vi "Interface Browser.vi"(5 "Caller Window Bounds":T1, 7 "Name (\"\" to Use Uuid)":string=".interface-browser", 10 "Init State (\"Macro: Initialize\")":string="Macro: Initialize") -> ()   [LabVIEW 2017]
uses:
  <vilib>/Utility/miscctls.llb/LVRectTypeDef.ctl
  Def-FilterOption.ctl
  <vilib>/Utility/miscctls.llb/LVPoint32TypeDef.ctl
  Def-TreeData.ctl
  <vilib>/Utility/miscctls.llb/LVPointTypeDef.ctl
  AdvanceAPI/CSM - Revert Arguments-Safe String.vi
  AdvanceAPI/CSM - Break Down Multiple States String.vi
  AdvanceAPI/CSM - Compact Multiple States.vi
  AdvanceAPI/CSM - Make String Arguments Safe.vi
  AdvanceAPI/CSM - Keywords.vi
  _Polymophic/Add State(s) to Queue By BOOL(Element).vi
  _csmHelper/API/Destroy.vi
  _csmHelper/API/Stop Undo.vi
  _csmHelper/API/Open Block Diagram.vi
  _csmHelper/API/Connect Paired Tunnels.vi
  _csmHelper/API/Add State Frame.vi
  _csmHelper/API/Start Undo.vi
  _csmHelper/API/Create From VI Reference.vi
  _csmHelper/API/Open Front Panel.vi
  _Polymophic/CSM - Filter Duplicated Lines.vi
  Communicable State Machine.lvlib
  _ui/csm-ui-support.lvlib
  _csmHelper/API with lvcsm Support/CSM-Helper API with lvcsm Support.lvlib
  _interfacebrowser/interfacebrowser.lvlib
  _csmHelper/CSM-Helper.lvclass
  _csmHelper/lvcsmFile/lvcsm File Support.lvlib
  _Shared/CSM Shared.lvlib
panel:
  in  "Option:Online Only":bool
  in  "Option:All-CSM-VIs":bool
  in  "Scan Project":bool
  in  "Refresh":bool
  in  "Fast Forward":bool
  in  "Fast Reverse":bool
  in  "Skip to Beginning":bool
  in  "Skip to End":bool
  in  "Stop":bool
  in  "Play":bool
  in  "Open":bool
  in  "Refresh lvcsm Cache":bool
  in  "Filter":string
  in  "FilterOption":T2
  in  "Reset Filter":bool
  in  "MainTree":string[](tree)
  in  "Option:Sync Filter On States":bool
  in  "Zoom Factor":dbl(slide)=0.1 min=0.1 max=1.0 step=0.001 scale=0.1..1.0
  in  "Interface-Filter":enum16{"API-Only", "UserDef States", "All"}(ring)=enum."UserDef States"
  in  "CSM-States":i32[](listbox) caption="Interface"
  in  "CSM-Status":i32[](listbox) caption="Status"
  out "StateInfo@Image":string
  out "Preview":picture
  out "String":string
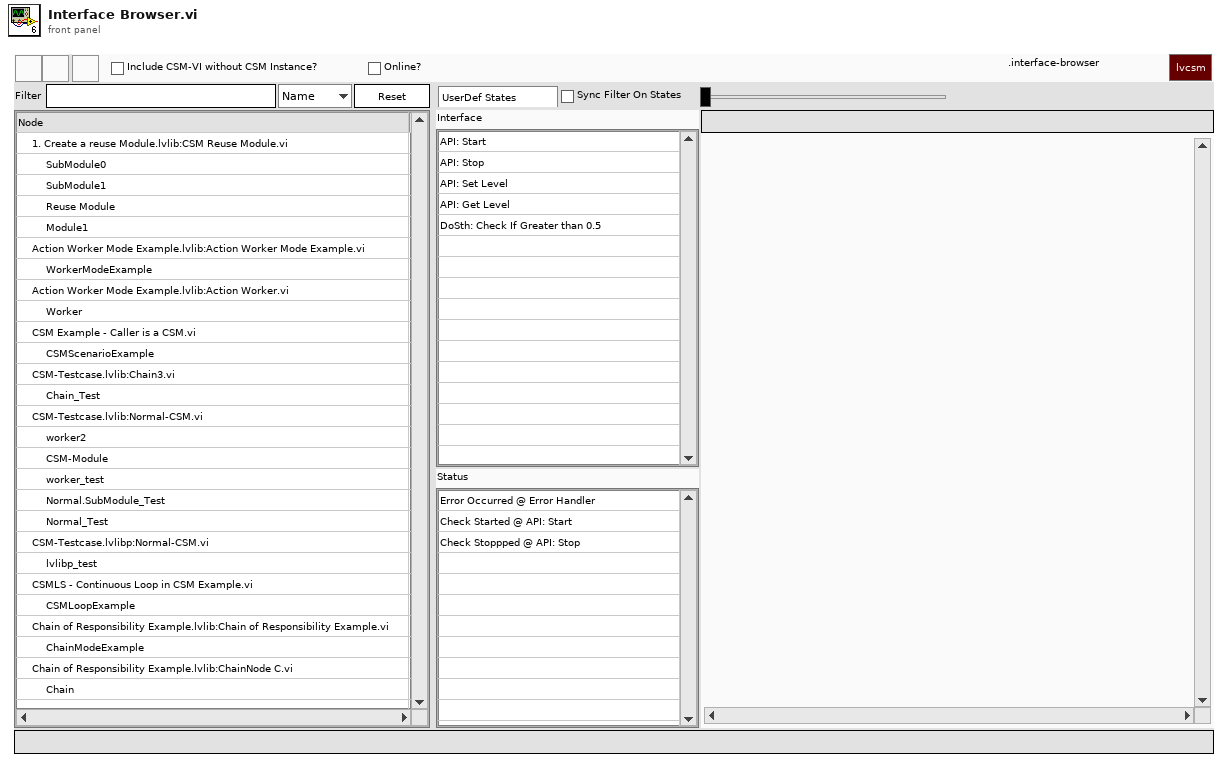
[diagram p1: front panel]
types:
  T1 = typedef "LVRectTypeDef.ctl" = cluster{"Left":i16, "Top":i16, "Right":i16, "Bottom":i16}
  T2 = typedef "Def-FilterOption.ctl" = enum16{"Name", "State"}
  T3 = enum32{"Invalid", "Standard", "Closed", "Hidden", "Minimized", "Maximized"}
  T4 = enum32{"invalid app kind", "Development System", "Run Time System", "Student Edition", "Embedded LabVIEW", "Evaluation", "Custom"}
  T5 = typedef "LVPointTypeDef.ctl" = cluster{"Horizontal":i16, "Vertical":i16}
  T6 = cluster{"Opton:All-CSM-VIs":bool, "Option:Online Only":bool}
  T7 = typedef "Communicable State Machine.lvlib/_CSM_Response Source Message.ctl" = cluster{"‘State":string, "’Arguments":string, "’Error":errorcluster}
  T8 = cluster{"Current VI Reference":refnum<vi>, "Close Panel on Exit?":bool}
  T9 = typedef "Def-TreeData.ctl" = cluster{"Type":string[], "Table":string[][]}
  T10 = cluster{"Core":cluster{"Current VI Reference":refnum<vi>, "Close Panel on Exit?":bool}, "BD-IMG":picture, "Tree":T9}
  T11 = typedef "LVPoint32TypeDef.ctl" = cluster{"Horizontal":i32, "Vertical":i32}
  T12 = cluster{"your data":bool, "PreviewMouseDown":bool, "PreviewMouseDownCoords":T11, "PreviewMouseDownOrigin":T11}
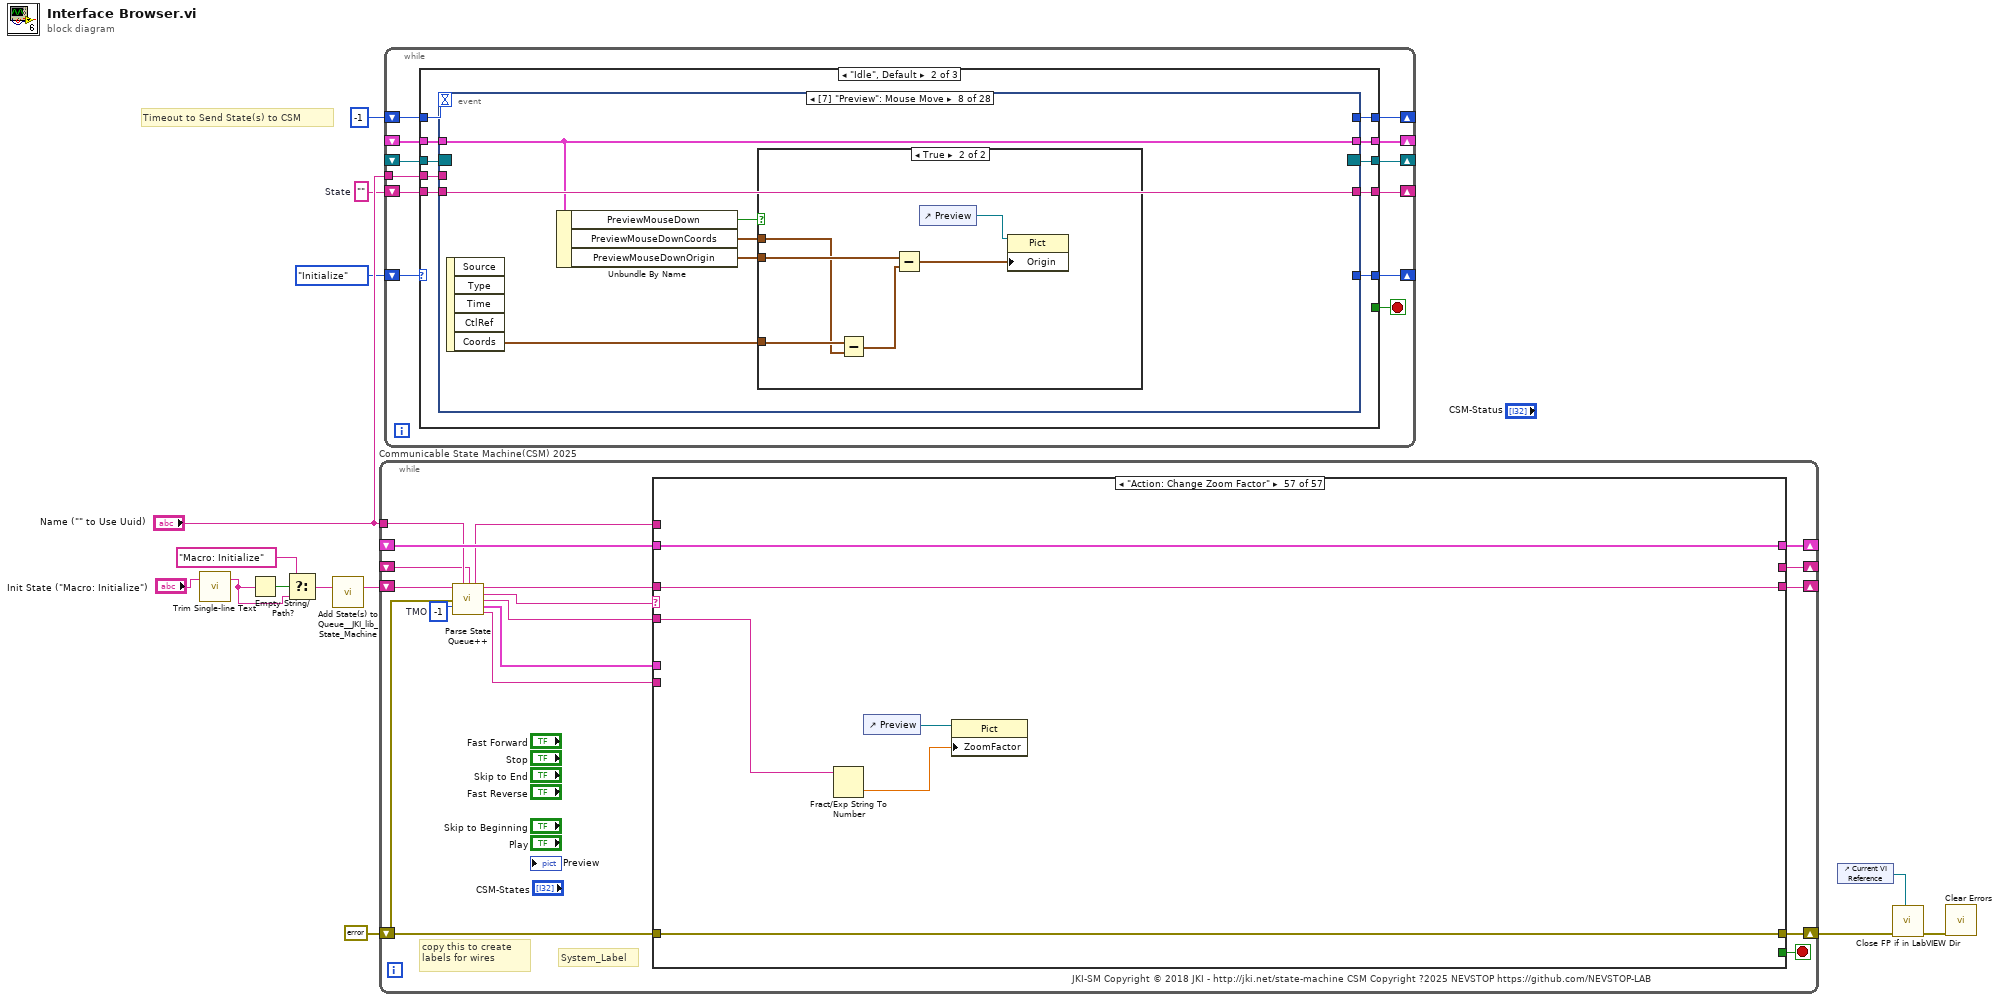
[diagram p0: block diagram]
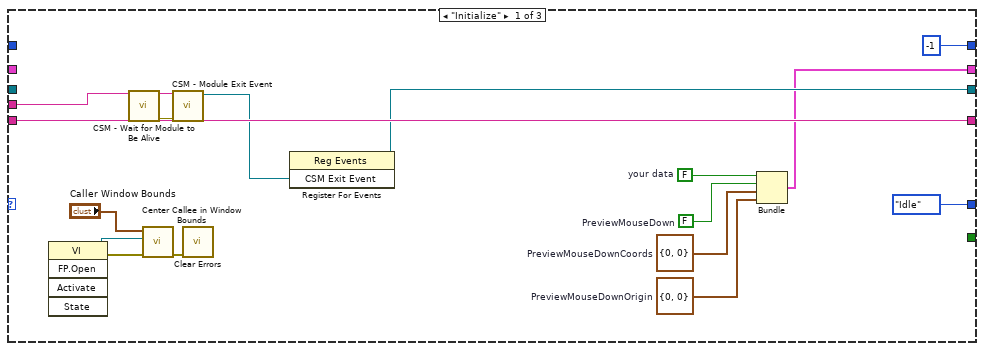
[diagram p2: hidden frame]
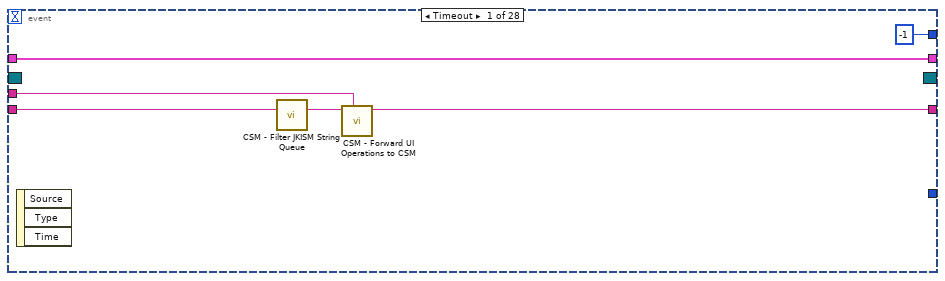
[diagram p3: hidden frame]
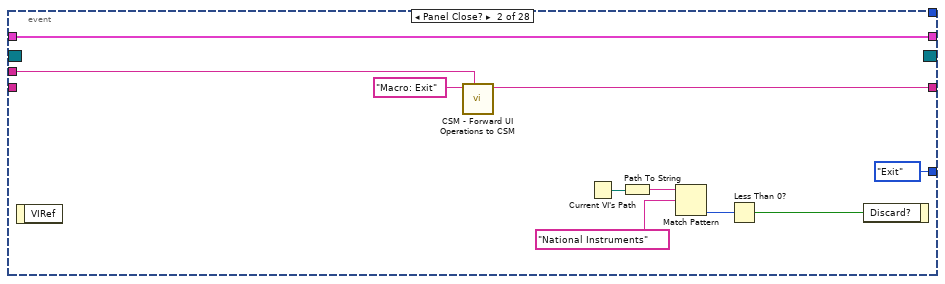
[diagram p4: hidden frame]
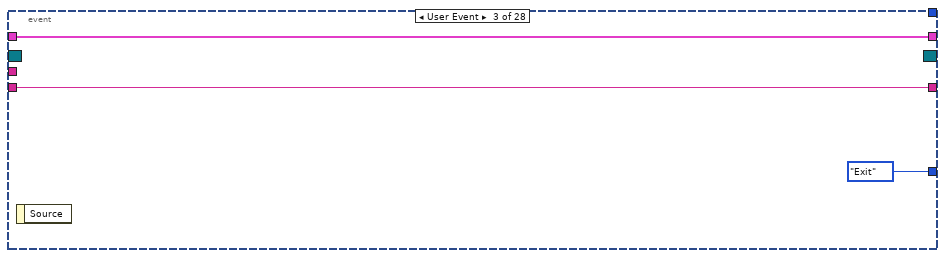
[diagram p5: hidden frame]
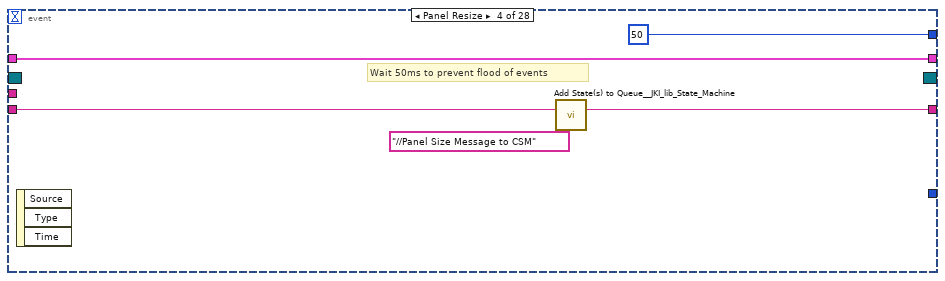
[diagram p6: hidden frame]
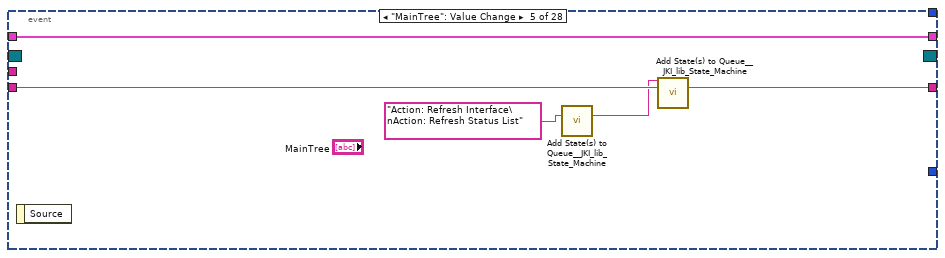
[diagram p7: hidden frame]
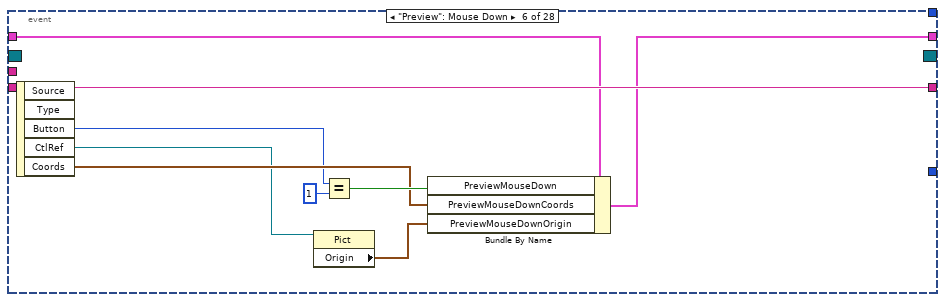
[diagram p8: hidden frame]
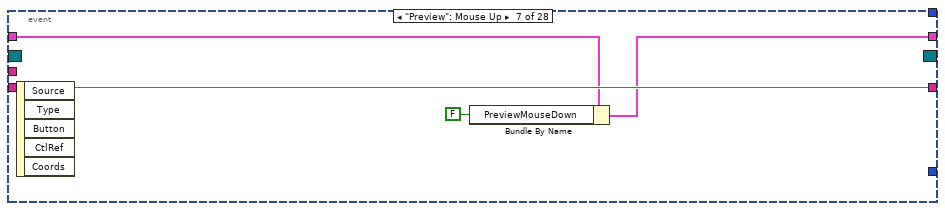
[diagram p9: hidden frame]
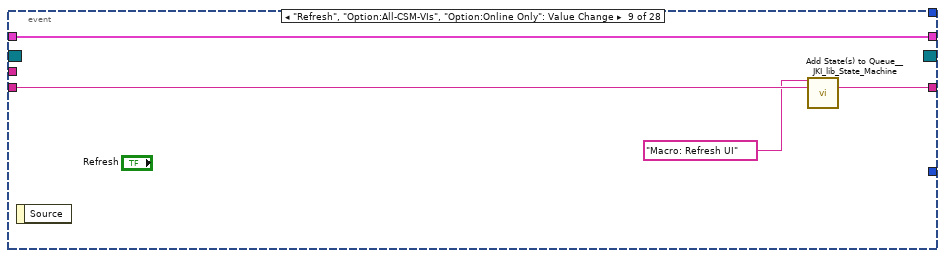
[diagram p11: hidden frame]
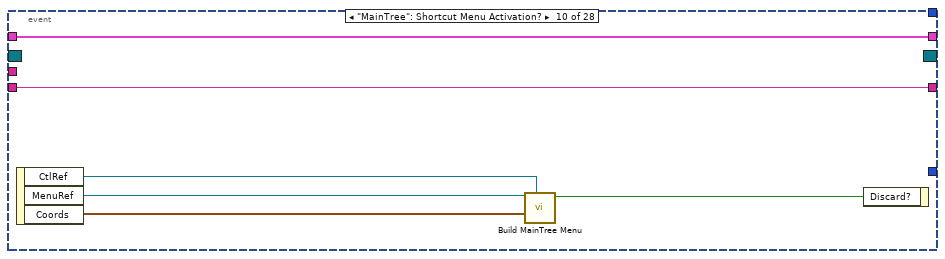
[diagram p12: hidden frame]
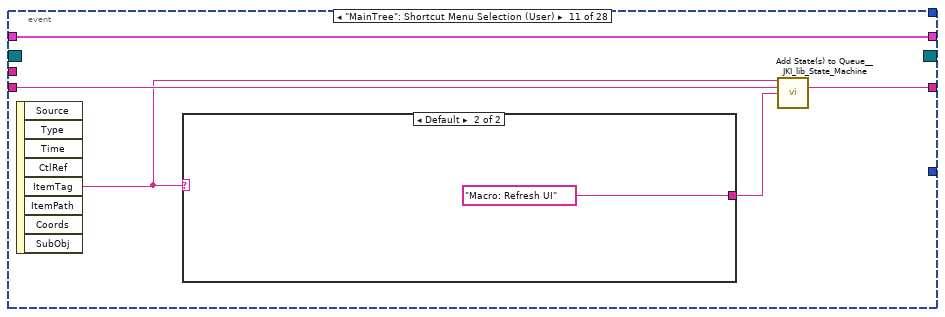
[diagram p13: hidden frame]
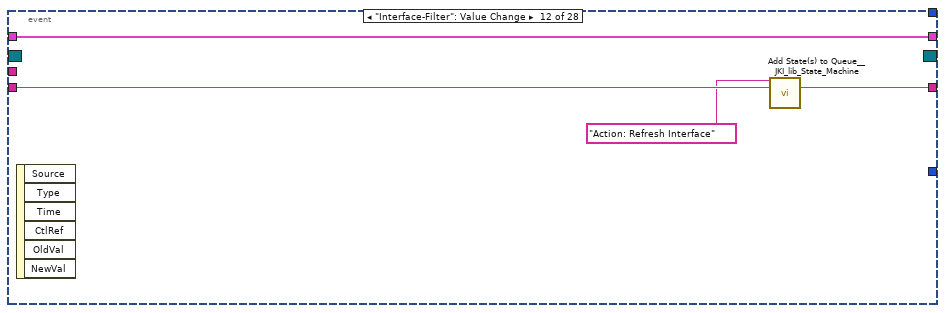
[diagram p15: hidden frame]
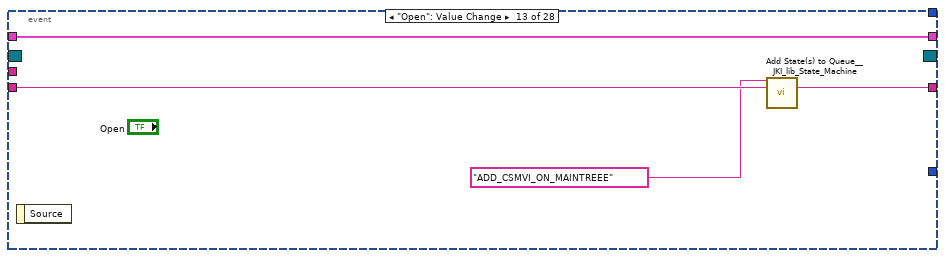
[diagram p16: hidden frame]
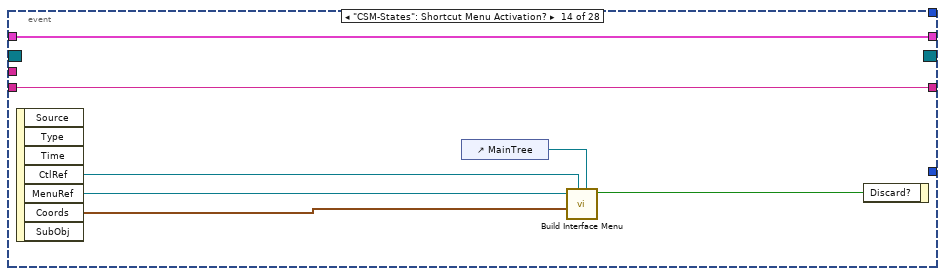
[diagram p17: hidden frame]
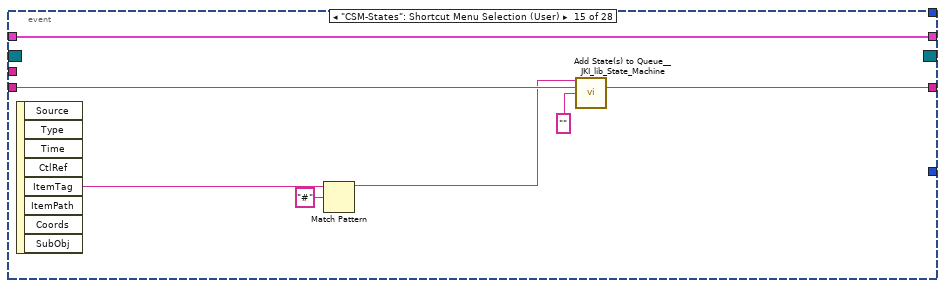
[diagram p18: hidden frame]
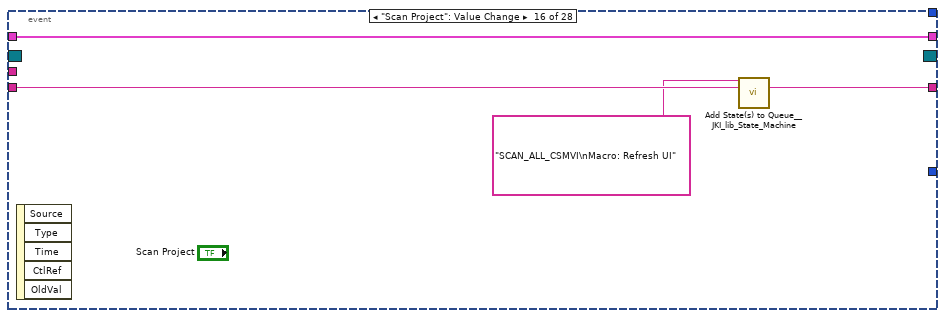
[diagram p19: hidden frame]
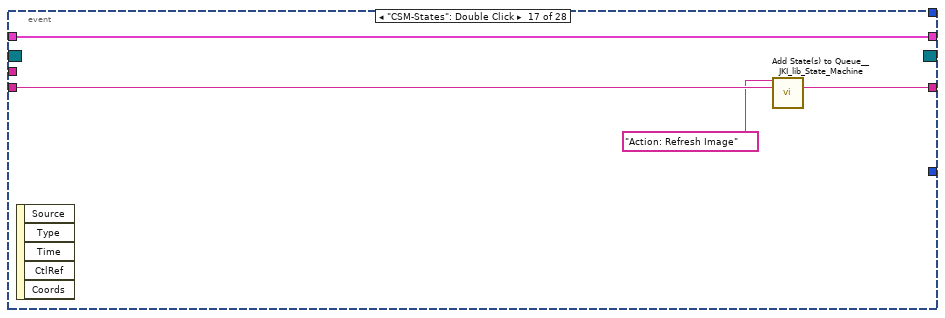
[diagram p20: hidden frame]
diagram:
  w12 = ""  # State
  # "Timeout to Send State(s) to CSM"
  n1 = call "Trim Single-line Text.vi"("single-line text"="Init State (\"Macro: Initialize\")") -> ("trimed text"=w5:string)  [unwired: 2 in]
  n2 = Empty String/Path?(string/path=w5) -> (empty?=w7:bool)
  n3 = Select(t="Macro: Initialize", s=w7, f=w5) -> (s? t:f=w6:string)
  n4 = call <vilib>:"Add State(s) to Queue__JKI_lib_State_Machine.vi"("State(s) in (\"\")"=w6) -> ("States Out"=w8:string)  [unwired: 14 in]
  n5 = while "Communicable State Machine(CSM) 2025" {
    shift-right: [w26] -> _
    shift-left: _ -> [w25]
    shift-right: [w29] -> w1
    shift-left: errorcluster {"status"=FALSE, "code"=0, "source"=""} ("error out") -> [w15]
    shift-right: [w28] -> _
    shift-left: w8 -> [w30]
    tunnel: "Name (\"\" to Use Uuid)" -> [w22]
    shift-right: [w23] -> _
    shift-left: _ -> [w17]
    stop <- w27 stop-if-true
    w24 = -1  # TMO
    # "JKI-SM Copyright © 2018 JKI - http://jki.net/state-machine CSM Copyright ?2025 NEVSTOP https://github.com/NEVSTOP-LAB"
    # "copy this to create labels for wires"
    # "System_Label"
    n6 = call "Parse State Queue++.vi"("State Queue"=w30, "Name (\"\" to Use UUID)"=w22, "Response Arguments"=w17, "Previous Error"=w15, "Dequeue (1 ms)"=w24) -> ("Name Used"=w16:string, "Remaining States"=w31:string, "Current State"=w18:string, "Arguments"=w19:string, "Additional Information"=w20:T7, "Source CSM"=w21:string)  [unwired: 5 in]
    n7 = case shown="\"Action: Change Zoom Factor\"" w18 {
      selector: w18 -> [_ _ _ w42 _ _ _ _ _ _ _ _ _ _ _ _ _ _ _ _ _ _ _ _ _ _ _ _ _ _ _ _ _ _ _ _ _ _ _ _ _ _ _ _ _ _ _ _ _ _ _ _ _ _ _ _ _]
      tunnel: w31 -> [w32 w35 w38 w46 w51 w57 w80 w86 w92 w102 w109 w121 w125 w128 w134 w149 w155 w158 w162 w166 w172 w174 w184 w198 w205 w222 w234 w255 w276 w289 w303 w317 w334 w336 w379 w404 w416 w428 w437 w458 w460 w465 w470 w482 w502 w514 w525 w536 w543 w559 w576 w615 w641 w656 w677 w697 w727]
      tunnel: w19 -> [_ _ _ _ _ w56 w76 w83 w89 w96 _ _ _ _ _ _ _ _ _ _ _ _ _ _ _ _ _ _ _ _ _ _ _ _ _ _ _ _ _ _ _ _ _ w478 w493 _ _ _ _ _ _ _ w637 _ _ _ w724]
      tunnel: w25 -> [w33 w34 w36 w44 w50 w62 w78 w84 w90 w100 w108 w115 w123 w126 _ w148 w150 w156 w160 w164 w170 w173 w183 w197 w208 w221 w233 w254 w275 w288 w302 w316 w333 w346 w384 w406 w418 w430 w436 w457 w462 w467 w469 w481 w501 w512 w523 w534 w544 w550 w574 w613 w640 w666 w686 w696 w726]
      tunnel: [_ _ _ w39 w52 errorcluster {"status"=FALSE, "code"=0, "source"=""} ("error out") w73 w81 w87 w103 _ _ _ _ _ _ w151 _ _ _ _ w175 w178 w193 _ w213 w226 w240 w256 w277 w291 w310 w332 w347 w383 w398 w412 w424 w435 w456 w463 w468 _ w472 w496 _ w516 _ w542 _ _ _ w639 _ _ w687 w728] -> w29
      tunnel: w15 -> [_ _ _ w40 w52 w60 w74 w82 w88 _ _ _ _ _ _ _ w152 _ _ _ _ w175 _ _ _ _ _ _ _ _ _ _ _ w347 _ _ _ _ _ _ w463 w468 _ _ _ _ _ _ _ _ _ _ _ _ _ _ w728]
      tunnel: [w32 w35 w37 w45 w51 w58 w79 w85 w91 w101 w109 w120 w124 w127 w133 w149 w154 w157 w161 w165 w171 w174 w184 w198 w206 w222 w234 w255 w276 w289 w303 w317 w334 w337 w380 w405 w417 w429 w437 w458 w461 w466 w470 w482 w502 w513 w524 w535 w545 w558 w575 w614 w641 w657 w678 w697 w727] -> w28
      tunnel: [_ _ _ _ _ _ TRUE _ _ _ _ _ TRUE _ _ _ _ _ _ _ _ _ _ _ _ _ _ _ _ _ _ _ _ _ _ _ _ _ _ _ _ _ _ _ _ _ _ _ _ _ _ _ _ _ _ _ _] -> w27
      tunnel: [w33 w34 w36 w44 w50 w62 w78 w84 w90 w99 w108 w119 w123 w126 w132 w148 w150 w156 w160 w164 w170 w173 w183 w197 w208 w221 w233 w254 w275 w288 w302 w316 w333 w346 w384 w406 w418 w430 w436 w457 w462 w467 w469 w481 w501 w512 w523 w533 w544 w550 w574 w613 w640 w666 w686 w696 w726] -> w26
      tunnel: w21 -> [_ _ _ _ _ w55 _ _ _ w97 _ _ _ _ _ _ _ _ _ _ _ _ _ _ _ _ _ _ _ _ _ _ _ _ _ _ _ _ w432 _ _ _ _ _ _ _ _ _ _ _ _ _ _ _ _ _ _]
      tunnel: w20 -> [_ _ _ _ _ w54 _ _ _ w98 _ _ _ _ _ _ _ _ _ _ _ _ _ _ _ _ _ _ _ _ _ _ _ _ _ _ _ _ _ _ _ _ _ _ _ _ _ _ _ _ _ _ _ _ _ _ _]
      tunnel: [_ _ _ "" w47 _ _ _ _ _ _ _ _ _ _ _ _ _ _ _ _ _ _ _ _ _ _ _ _ _ _ _ _ _ _ _ _ _ _ _ _ _ _ _ _ _ _ _ _ _ _ _ _ _ _ _ _] -> w23
      tunnel: w16 -> [_ _ _ w41 _ _ w75 _ _ _ _ _ _ _ _ _ _ _ _ _ _ _ _ _ _ _ _ _ _ _ _ _ _ _ _ _ _ _ _ _ _ _ _ _ _ _ _ _ w539 _ _ _ _ _ _ _ _]
      frame "", "Idle" {
      }
      frame "CSM Documentation" {
      }
      frame "---------- Core ----------" {
        n8 = call <vilib>:"Add State(s) to Queue__JKI_lib_State_Machine.vi"("State(s) in (\"\")"=w38) -> ("States Out"=w37:string)  [unwired: 14 in]
      }
      frame Default {
        n9 = call "CSM Unhandled State Error.vi"("error in (no error)"=w40, "Undefined State"=w42, "CSM Name"=w41) -> ("error out"=w39:errorcluster)  [unwired: 8 in]
        n10 = call <vilib>:"Add State(s) to Queue__JKI_lib_State_Machine.vi"("State(s) in (\"\")"=w46) -> ("States Out"=w45:string)  [unwired: 14 in]
      }
      frame "VI Reference" {
        n11 = Unbundle By Name(w50) -> ("Core"=w49:T8)
        n12 = Unbundle By Name(w49) -> ("Current VI Reference"=w48:refnum<vi>)
        n13 = call "CSM - Convert Data to HexStr.vi"("Variant"=w48) -> ("HEX String (0-9,A-F)"=w47:string)  [unwired: 8 in]
      }
      frame "Error Handler" {
        # "Clear error"
        n14 = case shown="Error" w60 {
          selector: w60 -> [_ w67]
          tunnel: [w66 w69] -> w59
          tunnel: w57 -> [w66 w68]
          tunnel: w56 -> [w65 _]
          tunnel: w55 -> [_ _]
          tunnel: w54 -> [_ _]
          tunnel: [w64 w67] -> w53
          frame No Error {
            n15 = call "CSM - Convert Argument to Error.vi"("Argument"=w65) -> ("Error"=w64:errorcluster)  [unwired: 4 in]
            n16 = flat-sequence {
              tunnel: w64 -> [_]
              frame #0 {
              }
            }
          }
          frame Error {
            n17 = call "CSM - Convert Error to Argument.vi"("Error"=w67) -> ("Argument"=w71:string)  [unwired: 4 in]
            n18 = call <vilib>:"Build State String with Arguments__JKI_lib_State_Machine.vi"("Arguments (\"\")"=w71, "State"="Error Occurred" ("Status with Arguments")) -> ("State with Arguments"=w70:string)  [unwired: 4 in]
            n19 = call "CSM - Broadcast Status Change.vi"("Status With Arguments"=w70, "State Queue"=w68) -> ("Remaining States"=w69:string)  [unwired: 13 in]
          }
        }
        n20 = call <vilib>:"Simple Error Handler.vi"("error in (no error)"=w53) -> ()  [unwired: 4 in, 5 out]
        n21 = call <vilib>:"Add State(s) to Queue__JKI_lib_State_Machine.vi"("State(s) in Front (\"\")"="// Post Error States", "State(s) in (\"\")"=w59) -> ("States Out"=w58:string)  [unwired: 13 in]
      }
      frame "Critical Error" {
        n22 = call "CSM Critical Error.vi"("error in (no error)"=w74, "Arugments (As Reason)"=w76, "CSM Name"=w75) -> ("error out"=w73:errorcluster)  [unwired: 8 in]
        n23 = call <vilib>:"Add State(s) to Queue__JKI_lib_State_Machine.vi"("State(s) in (\"\")"=w80) -> ("States Out"=w79:string)  [unwired: 14 in]
      }
      frame "Target Timeout Error" {
        n24 = call "CSM Target Timeout Error.vi"("error in (no error)"=w82, "Arguments (As CSM Name)"=w83) -> ("error out"=w81:errorcluster)  [unwired: 9 in]
        n25 = call <vilib>:"Add State(s) to Queue__JKI_lib_State_Machine.vi"("State(s) in (\"\")"=w86) -> ("States Out"=w85:string)  [unwired: 14 in]
      }
      frame "Target Error" {
        n26 = call "CSM Target Error.vi"("error in (no error)"=w88, "Arguments (As CSM Name)"=w89) -> ("error out"=w87:errorcluster)  [unwired: 9 in]
        n27 = call <vilib>:"Add State(s) to Queue__JKI_lib_State_Machine.vi"("State(s) in (\"\")"=w92) -> ("States Out"=w91:string)  [unwired: 14 in]
      }
      frame "Async Response", "Response" {
        n28 = Unbundle(w98) -> ("‘State"=w95:string, "’Arguments"=w94:string, "’Error"=w93:errorcluster)
        n29 = case shown="Default" w95 {
          tunnel: [w104] -> w101
          tunnel: w102 -> [w105]
          tunnel: [w107] -> w99
          tunnel: w100 -> [w107]
          tunnel: [w106] -> w103
          tunnel: w93 -> [w106]
          tunnel: w97 -> [_]
          tunnel: w96 -> [_]
          tunnel: w94 -> [_]
          frame Default {
            n30 = call <vilib>:"Add State(s) to Queue__JKI_lib_State_Machine.vi"("State(s) in (\"\")"=w105) -> ("States Out"=w104:string)  [unwired: 14 in]
          }
        }
      }
      frame "Async Message Posted" {
      }
      frame "Initialize Core Data" {
        # "originally closed?"
        # "exe?"
        # "If panel starts closed or is an EXE, then close it when we exit"
        n31 = control-ref of="Current VI Reference"() -> (w113:refnum<vi>)
        n32 = property class="VI"() -> ("FP.State"=w112:T3)  [unwired: 2 in, 2 out]
        n33 = property class="App"() -> ("App.Kind"=w118:T4)  [unwired: 2 in, 2 out]
        n34 = Equal?(x=w112, y=T3."Closed" ("Front Panel Window:State")) -> (x = y?=w110:bool)
        n35 = Equal?(x=w118, y=T4."Run Time System" ("Application:Kind")) -> (x = y?=w116:bool)
        n36 = Or(x=w110, y=w116) -> (x .or. y?=w114:bool)
        n37 = Bundle By Name(cluster=w115, "Core.Current VI Reference"=w113, "Core.Close Panel on Exit?"=w114) -> (w119:T10)
        n38 = call <vilib>:"Add State(s) to Queue__JKI_lib_State_Machine.vi"("State(s) in (\"\")"=w121) -> ("States Out"=w120:string)  [unwired: 14 in]
      }
      frame "Exit" {
        n39 = call <vilib>:"Add State(s) to Queue__JKI_lib_State_Machine.vi"("State(s) in (\"\")"=w125) -> ("States Out"=w124:string)  [unwired: 14 in]
      }
      frame "---------- Data ----------" {
        n40 = call <vilib>:"Add State(s) to Queue__JKI_lib_State_Machine.vi"("State(s) in (\"\")"=w128) -> ("States Out"=w127:string)  [unwired: 14 in]
      }
      frame "Data: Initialize" {
        w129 = T9 {"Type"=[], "Table"=[]}  # Tree
        w130 = picture data[5B]  # BD-IMG
        w131 = T8 {"Current VI Reference"=refnum, "Close Panel on Exit?"=FALSE}  # Core
        n41 = Bundle("Core"=w131, "BD-IMG"=w130, "Tree"=w129) -> (w132:T10)  [unwired: 1 in]
        n42 = call <vilib>:"Add State(s) to Queue__JKI_lib_State_Machine.vi"("State(s) in (\"\")"=w134) -> ("States Out"=w133:string)  [unwired: 14 in]
      }
      frame "Data: Update Indicators" {
        n43 = property class="App"() -> ("Project.ActiveProject"=w144:refnum<vi>)  [unwired: 2 in, 2 out]
        n44 = property class="Project"(reference=w144) -> ("Path"=w145:path)  [unwired: 1 in, 2 out]
        n45 = Strip Path(path=w145) -> (stripped path=w141:path)  [unwired: 1 out]
        n46 = local write "Preview"(picture data[5B] ("2D Picture 2")) -> ()
        n47 = local write "FilterOption"(Def-FilterOption."Name" ("FilterOption")) -> ()
        n48 = property on="Preview" class="Pict"("Origin"=T5 {"Horizontal"=0, "Vertical"=0}) -> ()  [unwired: 2 in, 2 out]
        n49 = Path To String(path=w141) -> (string=w140:string)
        n50 = call <vilib>:"Build State String with Arguments__JKI_lib_State_Machine.vi"("Arguments (\"\")"=w140, "State"="Interface Browser (CSM) ") -> ("State with Arguments"=w143:string)  [unwired: 4 in]
        n51 = property on="CSM-Status" class="LstBox (strict)"("Item Names"=string[] []) -> ()  [unwired: 2 in, 2 out]
        n52 = local write "Option:Sync Filter On States"(TRUE ("Option:Sync Filter On States")) -> ()
        n53 = local write "Zoom Factor"(0.7 ("Zoom Factor")) -> ()
        n54 = local write "Filter"("" ("Filter")) -> ()
        n55 = property class="VI"("Front Panel.Title"=w143) -> ()  [unwired: 2 in, 2 out]
      }
      frame "Data: Cleanup" {
        n56 = Unbundle By Name(w150) -> ("Core.Current VI Reference"=w153:refnum<vi>)
        n57 = Close Reference(reference=w153, error in (no error)=w152) -> (error out=w151:errorcluster)
        n58 = call <vilib>:"Add State(s) to Queue__JKI_lib_State_Machine.vi"("State(s) in (\"\")"=w155) -> ("States Out"=w154:string)  [unwired: 14 in]
      }
      frame "---------- Macro ----------" {
        n59 = call <vilib>:"Add State(s) to Queue__JKI_lib_State_Machine.vi"("State(s) in (\"\")"=w158) -> ("States Out"=w157:string)  [unwired: 14 in]
      }
      frame "Macro: Initialize" {
        n60 = call <vilib>:"Add State(s) to Queue__JKI_lib_State_Machine.vi"("State(s) in Front (\"\")"="Data: Initialize\nInitialize Core Data\nData: Update Indicators\nMacro: Refresh UI", "State(s) in (\"\")"=w162) -> ("States Out"=w161:string)  [unwired: 13 in]
      }
      frame "Macro: Refresh UI" {
        n61 = call <vilib>:"Add State(s) to Queue__JKI_lib_State_Machine.vi"("State(s) in Front (\"\")"="Action: Refresh(CSM-VI mode)\nAction: Refresh Symbol\nAction: Refresh Interface\nAction: Refresh Status List\nAction: Refresh Image\n", "State(s) in (\"\")"=w166) -> ("States Out"=w165:string)  [unwired: 13 in]
      }
      frame "Macro: Exit" {
        n62 = call <vilib>:"Add State(s) to Queue__JKI_lib_State_Machine.vi"("State(s) in Front (\"\")"="//Exit Sub-Modules ", "State(s) at Back (\"\")"="Data: Cleanup\nExit") -> ("States Out"=w168:string)  [unwired: 13 in]
        n63 = call <vilib>:"Add State(s) to Queue__JKI_lib_State_Machine.vi"("State(s) in Front (\"\")"=w168, "State(s) in (\"\")"=w172) -> ("States Out"=w171:string)  [unwired: 13 in]
      }
      frame "------ Menu Handler ------" {
      }
      frame "ADD_CSM_ON_CSMVI" {
        n64 = control-ref of="MainTree"() -> (w182:refnum<vi>)
        n65 = property class="Tree (strict)"(reference=w182) -> ("Value"=w181:string[])  [unwired: 1 in, 2 out]
        n66 = call "CSM Module Name"() -> ("CSM Module"=w179:string, "OK"=w177:bool)  [unwired: 17 in, 1 out]
        n67 = Index Array(array=w181) -> (element=w180:string)  [unwired: 1 in]
        n68 = call <vilib>:"Trim Whitespace.vi"("string"=w179) -> ("trimmed string"=w176:string)  [unwired: 1 in]
        n69 = case shown="True" w177 {
          tunnel: w180 -> [_ w187]
          tunnel: w176 -> [_ w186]
          tunnel: [_ w185] -> w178
          frame False {
          }
          frame True {
            n70 = call "Add CSM Module.vi"("CSM-VI"=w187, "CSM Name"=w186) -> ("error out"=w185:errorcluster)  [unwired: 9 in]
          }
        }
      }
      frame "ADD_CSM_ON_CSM" {
        n71 = control-ref of="MainTree"() -> (w196:refnum<vi>)
        n72 = property class="Tree (strict)"(reference=w196) -> ("Value"=w195:string[])  [unwired: 1 in, 2 out]
        n73 = Index Array(array=w195) -> (element=w190:string)  [unwired: 1 in]
        n74 = call "CSM Module Name2"() -> ("CSM Module"=w194:string, "OK"=w192:bool)  [unwired: 17 in, 1 out]
        n75 = Match Pattern(string=w190, regular expression="/") -> (before substring=w189:string)  [unwired: 1 in, 3 out]
        n76 = call <vilib>:"Trim Whitespace.vi"("string"=w194) -> ("trimmed string"=w191:string)  [unwired: 1 in]
        n77 = case shown="True" w192 {
          tunnel: w189 -> [_ w201]
          tunnel: w191 -> [_ w200]
          tunnel: [_ w199] -> w193
          frame False {
          }
          frame True {
            n78 = call "Add CSM Module.vi"("CSM-VI"=w201, "CSM Name"=w200) -> ("error out"=w199:errorcluster)  [unwired: 9 in]
          }
        }
      }
      frame "ADD_CSMVI_ON_MAINTREEE" {
        n79 = call "File Dialog"("pattern (all files)"="*.vi") -> ("selected path"=w203:path, "error out"=w204:errorcluster)  [unwired: 11 in, 2 out]
        n80 = case shown="Error" w204 {
          selector: w204 -> [w211 _]
          tunnel: w203 -> [w212 _]
          tunnel: ["Macro: Refresh UI" ("State(s) in Front (\"\")") _] -> w202
          frame No Error {
            n81 = call "Add CSM-VI.vi"("error in (no error)"=w211, "CSM-VI"=w212) -> ("error out"=w209:errorcluster)  [unwired: 9 in]
            n82 = call <vilib>:"Simple Error Handler.vi"("error in (no error)"=w209) -> ()  [unwired: 4 in, 5 out]
          }
          frame Error {
          }
        }
        n83 = call <vilib>:"Add State(s) to Queue__JKI_lib_State_Machine.vi"("State(s) in Front (\"\")"=w202, "State(s) in (\"\")"=w205) -> ("States Out"=w206:string)  [unwired: 13 in]
      }
      frame "RM_CSM_ON_CSM" {
        n84 = control-ref of="MainTree"() -> (w220:refnum<vi>)
        n85 = property class="Tree (strict)"(reference=w220) -> ("Value"=w219:string[])  [unwired: 1 in, 2 out]
        n86 = Index Array(array=w219) -> (element=w218:string)  [unwired: 1 in]
        n87 = Two Button Dialog(message="Are you sure to remove it?") -> (T button?=w214:bool)  [unwired: 2 in]
        n88 = Match Pattern(string=w218, regular expression="/") -> (after substring=w215:string)  [unwired: 1 in, 3 out]
        n89 = case shown="True" w214 {
          tunnel: w215 -> [_ w224]
          tunnel: [_ w223] -> w213
          frame False {
          }
          frame True {
            n90 = call "Delete CSM Module.vi"("CSM Name"=w224) -> ("error out"=w223:errorcluster)  [unwired: 10 in]
          }
        }
      }
      frame "RM_CSMVI_ON_CSMVI" {
        n91 = control-ref of="MainTree"() -> (w232:refnum<vi>)
        n92 = property class="Tree (strict)"(reference=w232) -> ("Value"=w231:string[])  [unwired: 1 in, 2 out]
        n93 = Index Array(array=w231) -> (element=w230:string)  [unwired: 1 in]
        n94 = Two Button Dialog(message="Are you sure to remove it?") -> (T button?=w227:bool)  [unwired: 2 in]
        n95 = Match Pattern(string=w230, regular expression="/") -> (before substring=w225:string)  [unwired: 1 in, 3 out]
        n96 = case shown="True" w227 {
          tunnel: w225 -> [_ w236]
          tunnel: [_ w235] -> w226
          frame False {
          }
          frame True {
            n97 = call "Delete CSM-VI.vi"("CSM Name"=w236) -> ("error out"=w235:errorcluster)  [unwired: 10 in]
          }
        }
      }
      frame "OPEN_CSMVI_ON_CSM", "OPEN_CSMVI_ON_CSMVI" {
        n98 = control-ref of="MainTree"() -> (w253:refnum<vi>)
        n99 = property class="Tree (strict)"(reference=w253) -> ("Value"=w252:string[])  [unwired: 1 in, 2 out]
        n100 = Index Array(array=w252) -> (element=w251:string)  [unwired: 1 in]
        n101 = Match Pattern(string=w251, regular expression="/") -> (before substring=w249:string)  [unwired: 1 in, 3 out]
        n102 = call "Read CSM-VI Info.vi"("CSM Name"=w249) -> ("Cluster 2"=w248:cluster{"Path":path})  [unwired: 9 in, 1 out]
        n103 = Unbundle By Name(w248) -> ("Path"=w238:path)
        n104 = Path To String(path=w238) -> (string=w237:string)
        n105 = call "lvcsm String to Path.vi"("Common Path"=w237) -> ("Path"=w239:path)  [unwired: 10 in]
        n106 = Open VI Reference(vi path=w239, options=2) -> (vi reference=w246:refnum<vi>, error out=w245:errorcluster)  [unwired: 4 in]
        n107 = call-poly "CSM-Helper API.vi"("error in (no error)"=w245, "VI"=w246) -> ("error out"=w243:errorcluster, "CSM-Helper.lvclass"=w244:refnum<class "CSM-Helper.lvclass">)  [unwired: 8 in]
        n108 = call-poly "CSM-Helper API.vi"("error in (no error)"=w243, "CSM-Helper in"=w244) -> ("error out"=w241:errorcluster, "CSM-Helper out"=w242:refnum<class "CSM-Helper.lvclass">)  [unwired: 8 in]
        n109 = call-poly "CSM-Helper API.vi"("error in (no error)"=w241, "CSM-Helper in"=w242) -> ("error out"=w240:errorcluster)  [unwired: 8 in, 1 out]
      }
      frame "EXPLORER_TO_FOLDER_ON_CSMVI" {
        n110 = control-ref of="MainTree"() -> (w274:refnum<vi>)
        n111 = property class="Tree (strict)"(reference=w274) -> ("Value"=w273:string[])  [unwired: 1 in, 2 out]
        n112 = Index Array(array=w273) -> (element=w272:string)  [unwired: 1 in]
        n113 = Match Pattern(string=w272, regular expression="/") -> (before substring=w270:string)  [unwired: 1 in, 3 out]
        n114 = call "Read CSM-VI Info.vi"("CSM Name"=w270) -> ("Cluster 2"=w269:cluster{"Path":path})  [unwired: 9 in, 1 out]
        n115 = Unbundle By Name(w269) -> ("Path"=w268:path)
        n116 = Path To String(path=w268) -> (string=w267:string)
        n117 = call "lvcsm String to Path.vi"("Common Path"=w267) -> ("Path"=w258:path)  [unwired: 10 in]
        n118 = File/Directory Info(path=w258) -> (directory=w264:bool, error out=w263:errorcluster)  [unwired: 1 in, 5 out]
        n119 = Compound Arithmetic op=OR(TRUE ("value"), invert w264) -> (w262:bool)
        n120 = Select(t="/select," ("format string"), s=w262, f="") -> (s? t:f=w261:string)
        n121 = Format Into String(format string="explorer %s\"%s\"", w261, w258) -> (resulting string=w265:string)  [unwired: 2 in, 1 out]
        n122 = call <vilib>:"System Exec.vi"("error in (no error)"=w263, "command line"=w265) -> ("error out"=w256:errorcluster)  [unwired: 6 in, 3 out]
      }
      frame "COPY_FULL_PATH_TO_CLIPBOARD" {
        n123 = control-ref of="MainTree"() -> (w287:refnum<vi>)
        n124 = property class="Tree (strict)"(reference=w287) -> ("Value"=w286:string[])  [unwired: 1 in, 2 out]
        n125 = Index Array(array=w286) -> (element=w285:string)  [unwired: 1 in]
        n126 = Match Pattern(string=w285, regular expression="/") -> (before substring=w283:string)  [unwired: 1 in, 3 out]
        n127 = call "Read CSM-VI Info.vi"("CSM Name"=w283) -> ("Cluster 2"=w282:cluster{"Path":path})  [unwired: 9 in, 1 out]
        n128 = Unbundle By Name(w282) -> ("Path"=w281:path)
        n129 = Path To String(path=w281) -> (string=w280:string)
        n130 = call "lvcsm String to Path.vi"("Common Path"=w280) -> ("Path"=w279:path)  [unwired: 10 in]
        n131 = Path To String(path=w279) -> (string=w278:string)
        n132 = invoke class="App" method="Clipboard.Write"("Param 0"=w278) -> (error out=w277:errorcluster)  [unwired: 3 in, 3 out]
      }
      frame "COPY_CNT_FOLDER_TO_CLIPBOARD" {
        n133 = control-ref of="MainTree"() -> (w301:refnum<vi>)
        n134 = property class="Tree (strict)"(reference=w301) -> ("Value"=w300:string[])  [unwired: 1 in, 2 out]
        n135 = Index Array(array=w300) -> (element=w299:string)  [unwired: 1 in]
        n136 = Match Pattern(string=w299, regular expression="/") -> (before substring=w297:string)  [unwired: 1 in, 3 out]
        n137 = call "Read CSM-VI Info.vi"("CSM Name"=w297) -> ("Cluster 2"=w296:cluster{"Path":path})  [unwired: 9 in, 1 out]
        n138 = Unbundle By Name(w296) -> ("Path"=w295:path)
        n139 = Path To String(path=w295) -> (string=w294:string)
        n140 = call "lvcsm String to Path.vi"("Common Path"=w294) -> ("Path"=w293:path)  [unwired: 10 in]
        n141 = Strip Path(path=w293) -> (stripped path=w290:path)  [unwired: 1 out]
        n142 = Path To String(path=w290) -> (string=w292:string)
        n143 = invoke class="App" method="Clipboard.Write"("Param 0"=w292) -> (error out=w291:errorcluster)  [unwired: 3 in, 3 out]
      }
      frame "GOTO_ON_CSMSTATE" {
        n144 = control-ref of="MainTree"() -> (w309:refnum<vi>)
        n145 = control-ref of="CSM-States"() -> (w314:refnum<vi>)
        n146 = property class="LstBox (strict)"(reference=w314) -> ("Item Names"=w315:string[], "Value"=w313:i32[])  [unwired: 1 in, 2 out]
        n147 = property class="Tree (strict)"(reference=w309) -> ("Value"=w308:string[])  [unwired: 1 in, 2 out]
        n148 = Index Array(array=w313) -> (element=w312:i32)  [unwired: 1 in]
        n149 = Index Array(array=w308) -> (element=w307:string)  [unwired: 1 in]
        n150 = Index Array(array=w315, index=w312) -> (element=w311:string)
        n151 = Match Pattern(string=w307, regular expression="/") -> (before substring=w305:string)  [unwired: 1 in, 3 out]
        n152 = call "Jump to CSM State.vi"("Type"=enum16{"CSM", "CSM-VI"}."CSM-VI", "State"=w311, "Name"=w305) -> ("error out"=w310:errorcluster)  [unwired: 8 in]
      }
      frame "GOTO_ON_CSMSTATUS" {
        (unwired) "@" ("string")
        n153 = control-ref of="CSM-Status"() -> (w322:refnum<vi>)
        n154 = property class="LstBox (strict)"(reference=w322) -> ("Item Names"=w325:string[], "Value"=w324:i32[])  [unwired: 1 in, 2 out]
        n155 = control-ref of="MainTree"() -> (w331:refnum<vi>)
        n156 = Index Array(array=w324) -> (element=w323:i32)  [unwired: 1 in]
        n157 = property class="Tree (strict)"(reference=w331) -> ("Value"=w330:string[])  [unwired: 1 in, 2 out]
        n158 = Index Array(array=w325, index=w323) -> (element=w321:string)
        n159 = Match Pattern(string=w321, regular expression="@") -> (after substring=w320:string)  [unwired: 1 in, 3 out]
        n160 = Index Array(array=w330) -> (element=w329:string)  [unwired: 1 in]
        n161 = call <vilib>:"Trim Whitespace.vi"("string"=w320) -> ("trimmed string"=w318:string)  [unwired: 1 in]
        n162 = Match Pattern(string=w329, regular expression="/") -> (before substring=w327:string)  [unwired: 1 in, 3 out]
        n163 = call "Jump to CSM State.vi"("Type"=enum16{"CSM", "CSM-VI"}."CSM-VI", "State"=w318, "Name"=w327) -> ("error out"=w332:errorcluster)  [unwired: 8 in]
      }
      frame "ADD_STATE_ON_CSMSTATE" {
        n164 = call "Add State"() -> ("State Name"=w345:string, "OK"=w338:bool, "error out"=w340:errorcluster)  [unwired: 17 in]
        n165 = Not(x=w340) -> (.not. x?=w341:bool)
        n166 = Empty String/Path?(string/path=w345) -> (empty?=w343:bool)
        n167 = And(x=w341, y=w338) -> (x .and. y?=w339:bool)
        n168 = Not(x=w343) -> (.not. x?=w344:bool)
        n169 = And(x=w344, y=w339) -> (x .and. y?=w342:bool)
        n170 = case shown="True" w342 {
          tunnel: w345 -> [_ w362]
          tunnel: [_ "RESCAN_INTERFACE_ON_CSMVI\nMacro: Refresh UI" ("State(s) in Front (\"\")")] -> w335
          frame False {
          }
          frame True {
            n171 = control-ref of="MainTree"() -> (w375:refnum<vi>)
            n172 = control-ref of="CSM-States"() -> (w376:refnum<vi>)
            n173 = property class="LstBox (strict)"(reference=w376) -> ("Item Names"=w377:string[])  [unwired: 1 in, 2 out]
            n174 = property class="Tree (strict)"(reference=w375) -> ("Value"=w374:string[])  [unwired: 1 in, 2 out]
            n175 = Index Array(array=w377) -> ()  [unwired: 1 in, 1 out]
            n176 = Index Array(array=w374) -> (element=w373:string)  [unwired: 1 in]
            n177 = Match Pattern(string=w373, regular expression="/") -> (before substring=w368:string)  [unwired: 1 in, 3 out]
            n178 = call "Read CSM-VI Info.vi"("CSM Name"=w368) -> ("error out"=w364:errorcluster, "Cluster 2"=w369:cluster{"Path":path})  [unwired: 9 in]
            n179 = Unbundle By Name(w369) -> ("Path"=w371:path)
            n180 = Path To String(path=w371) -> (string=w370:string)
            n181 = call "lvcsm String to Path.vi"("Common Path"=w370) -> ("Path"=w365:path)  [unwired: 10 in]
            n182 = Open VI Reference(vi path=w365, options=2, error in (no error)=w364) -> (vi reference=w366:refnum<vi>, error out=w367:errorcluster)  [unwired: 3 in]
            n183 = call-poly "CSM-Helper API.vi"("error in (no error)"=w367, "VI"=w366) -> ("error out"=w361:errorcluster, "CSM-Helper.lvclass"=w360:refnum<class "CSM-Helper.lvclass">)  [unwired: 8 in]
            n184 = call-poly "CSM-Helper API.vi"("error in (no error)"=w361, "CSM-Helper in"=w360) -> ("error out"=w359:errorcluster, "CSM-Helper out"=w358:refnum<class "CSM-Helper.lvclass">)  [unwired: 8 in]
            n185 = call-poly "CSM-Helper API.vi"("error in (no error)"=w359, "element"=w362, "CSM-Helper in"=w358) -> ("error out"=w351:errorcluster, "CSM-Helper out"=w350:refnum<class "CSM-Helper.lvclass">)  [unwired: 6 in, 1 out]
            n186 = call-poly "CSM-Helper API.vi"("error in (no error)"=w351, "CSM-Helper in"=w350) -> ("error out"=w348:errorcluster, "CSM-Helper out"=w349:refnum<class "CSM-Helper.lvclass">)  [unwired: 8 in]
            n187 = call-poly "CSM-Helper API.vi"("error in (no error)"=w348, "CSM-Helper in"=w349) -> ("error out"=w352:errorcluster, "CSM-Helper out"=w353:refnum<class "CSM-Helper.lvclass">)  [unwired: 8 in]
            n188 = call-poly "CSM-Helper API.vi"("error in (no error)"=w352, "CSM-Helper in"=w353) -> ("error out"=w357:errorcluster, "CSM-Helper out"=w356:refnum<class "CSM-Helper.lvclass">)  [unwired: 8 in]
            n189 = call-poly "CSM-Helper API.vi"("error in (no error)"=w357, "CSM-Helper in"=w356) -> ("error out"=w355:errorcluster)  [unwired: 8 in, 1 out]
            n190 = call <vilib>:"Simple Error Handler.vi"("error in (no error)"=w355) -> ()  [unwired: 4 in, 5 out]
          }
        }
        n191 = call <vilib>:"Add State(s) to Queue__JKI_lib_State_Machine.vi"("State(s) in Front (\"\")"=w335, "State(s) in (\"\")"=w336) -> ("States Out"=w337:string)  [unwired: 13 in]
      }
      frame "DELETE_STATE_ON_CSMSTATE" {
        n192 = Two Button Dialog(message="Are you sure?") -> (T button?=w381:bool)  [unwired: 2 in]
        n193 = case shown="True" w381 {
          tunnel: [_ w397] -> w383
          tunnel: [_ "RESCAN_INTERFACE_ON_CSMVI\nMacro: Refresh UI" ("State(s) in Front (\"\")")] -> w378
          frame False {
          }
          frame True {
            n194 = control-ref of="MainTree"() -> (w391:refnum<vi>)
            n195 = control-ref of="CSM-States"() -> (w395:refnum<vi>)
            n196 = property class="LstBox (strict)"(reference=w395) -> ("Item Names"=w396:string[], "Value"=w394:i32[])  [unwired: 1 in, 2 out]
            n197 = property class="Tree (strict)"(reference=w391) -> ("Value"=w390:string[])  [unwired: 1 in, 2 out]
            n198 = Index Array(array=w394) -> (element=w393:i32)  [unwired: 1 in]
            n199 = Index Array(array=w390) -> (element=w389:string)  [unwired: 1 in]
            n200 = Index Array(array=w396, index=w393) -> (element=w392:string)
            n201 = Match Pattern(string=w389, regular expression="/") -> (before substring=w387:string)  [unwired: 1 in, 3 out]
            n202 = call "Delete CSM State.vi"("Type"=enum16{"CSM", "CSM-VI"}."CSM-VI", "State"=w392, "Name"=w387) -> ("Error Out"=w397:errorcluster)  [unwired: 8 in]
          }
        }
        n203 = call <vilib>:"Add State(s) to Queue__JKI_lib_State_Machine.vi"("State(s) in Front (\"\")"=w378, "State(s) in (\"\")"=w379) -> ("States Out"=w380:string)  [unwired: 13 in]
      }
      frame "COPY_TO_CLIPBOARD_ON_CSMSTATE" {
        n204 = control-ref of="CSM-States"() -> (w402:refnum<vi>)
        n205 = property class="LstBox (strict)"(reference=w402) -> ("Item Names"=w403:string[], "Value"=w401:i32[])  [unwired: 1 in, 2 out]
        n206 = Index Array(array=w401) -> (element=w400:i32)  [unwired: 1 in]
        n207 = Index Array(array=w403, index=w400) -> (element=w399:string)
        n208 = invoke class="App" method="Clipboard.Write"("Param 0"=w399) -> (error out=w398:errorcluster)  [unwired: 3 in, 3 out]
        n209 = call <vilib>:"Add State(s) to Queue__JKI_lib_State_Machine.vi"("State(s) in (\"\")"=w404) -> ("States Out"=w405:string)  [unwired: 14 in]
      }
      frame "COPY_STATUS_TO_CLIPBOARD_ON_CSMSTATUS" {
        n210 = control-ref of="CSM-Status"() -> (w411:refnum<vi>)
        n211 = property class="LstBox (strict)"(reference=w411) -> ("Item Names"=w415:string[], "Value"=w414:i32[])  [unwired: 1 in, 2 out]
        n212 = Index Array(array=w414) -> (element=w413:i32)  [unwired: 1 in]
        n213 = Index Array(array=w415, index=w413) -> (element=w410:string)
        n214 = Match Pattern(string=w410, regular expression="@") -> (before substring=w408:string)  [unwired: 1 in, 3 out]
        n215 = call <vilib>:"Trim Whitespace.vi"("string"=w408) -> ("trimmed string"=w407:string)  [unwired: 1 in]
        n216 = invoke class="App" method="Clipboard.Write"("Param 0"=w407) -> (error out=w412:errorcluster)  [unwired: 3 in, 3 out]
        n217 = call <vilib>:"Add State(s) to Queue__JKI_lib_State_Machine.vi"("State(s) in (\"\")"=w416) -> ("States Out"=w417:string)  [unwired: 14 in]
      }
      frame "COPY_STATE_TO_CLIPBOARD_ON_CSMSTATUS" {
        n218 = control-ref of="CSM-Status"() -> (w423:refnum<vi>)
        n219 = property class="LstBox (strict)"(reference=w423) -> ("Item Names"=w427:string[], "Value"=w426:i32[])  [unwired: 1 in, 2 out]
        n220 = Index Array(array=w426) -> (element=w425:i32)  [unwired: 1 in]
        n221 = Index Array(array=w427, index=w425) -> (element=w422:string)
        n222 = Match Pattern(string=w422, regular expression="@") -> (after substring=w420:string)  [unwired: 1 in, 3 out]
        n223 = call <vilib>:"Trim Whitespace.vi"("string"=w420) -> ("trimmed string"=w419:string)  [unwired: 1 in]
        n224 = invoke class="App" method="Clipboard.Write"("Param 0"=w419) -> (error out=w424:errorcluster)  [unwired: 3 in, 3 out]
        n225 = call <vilib>:"Add State(s) to Queue__JKI_lib_State_Machine.vi"("State(s) in (\"\")"=w428) -> ("States Out"=w429:string)  [unwired: 14 in]
      }
      frame "SCAN_ALL_CSMVI" {
        n226 = case shown="\"\"" w432 {
          selector: w432 -> [w439 _]
          tunnel: [w438 w440] -> w431
          frame Default {
            n227 = call "lvcsm String to Path.vi"("Common Path"=w439) -> ("Path"=w438:path)  [unwired: 10 in]
          }
          frame "" {
            n228 = property class="App"() -> ("Project.ActiveProject"=w442:refnum<vi>)  [unwired: 2 in, 2 out]
            n229 = property class="Project"(reference=w442) -> ("Path"=w441:path)  [unwired: 1 in, 2 out]
            n230 = Strip Path(path=w441) -> (stripped path=w440:path)  [unwired: 1 out]
          }
        }
        n231 = Two Button Dialog(message="Scan for CSM Modules?") -> (T button?=w433:bool)  [unwired: 2 in]
        n232 = case shown="True" w433 {
          tunnel: [_ w445] -> w435
          tunnel: w431 -> [_ w444]
          frame False {
          }
          frame True {
            n233 = property class="VI"() -> ("Front Panel.PanelBounds"=w443:T1)  [unwired: 2 in, 2 out]
            n234 = call "Scan CSM-VI.vi"("Block Diagram Window:Window Bounds"=w443, "Root"=w444) -> ("Error Out"=w445:errorcluster)  [unwired: 9 in]
          }
        }
      }
      frame "RESCAN_INTERFACE_ON_CSMVI" {
        n235 = control-ref of="MainTree"() -> (w455:refnum<vi>)
        n236 = property class="Tree (strict)"(reference=w455) -> ("Value"=w454:string[])  [unwired: 1 in, 2 out]
        n237 = Index Array(array=w454) -> (element=w453:string)  [unwired: 1 in]
        n238 = Match Pattern(string=w453, regular expression="/") -> (before substring=w451:string)  [unwired: 1 in, 3 out]
        n239 = call "Read CSM-VI Info.vi"("CSM Name"=w451) -> ("error out"=w446:errorcluster, "Cluster 2"=w450:cluster{"Path":path})  [unwired: 9 in]
        n240 = Unbundle By Name(w450) -> ("Path"=w448:path)
        n241 = Path To String(path=w448) -> (string=w449:string)
        n242 = call "lvcsm String to Path.vi"("Common Path"=w449) -> ("Path"=w447:path)  [unwired: 10 in]
        n243 = call "Add CSM-VI.vi"("error in (no error)"=w446, "CSM-VI"=w447) -> ("error out"=w456:errorcluster)  [unwired: 9 in]
      }
      frame "CODEPREVIEW_ON_CSMSTATE" {
        n244 = call <vilib>:"Add State(s) to Queue__jki_lib_state_machine.vi"("State(s) in Front (\"\")"="Action: Refresh Image" ("State(s) in Front (\"\")"), "State(s) in (\"\")"=w460) -> ("States Out"=w461:string)  [unwired: 13 in]
      }
      frame "CODEPREVIEW_ON_CSMSTATUS" {
        n245 = call <vilib>:"Add State(s) to Queue__jki_lib_state_machine.vi"("State(s) in Front (\"\")"="Action: Refresh Image2" ("State(s) in Front (\"\")"), "State(s) in (\"\")"=w465) -> ("States Out"=w466:string)  [unwired: 13 in]
      }
      frame "---------- API ----------" {
      }
      frame "API: Set Current CSMVI" {
        n246 = control-ref of="MainTree"() -> (w480:refnum<vi>)
        n247 = property class="Tree (strict)"(reference=w480) -> (reference out=w474:refnum<vi>, error out=w473:errorcluster, "All Tags"=w479:string[])  [unwired: 1 in]
        n248 = for {
          tunnel: w479 -> [w490] mode=indexing
          tunnel: [w490] -> w476 mode=indexing if=w488
          n249 = Match Pattern(string=w490, regular expression="/") -> (offset past match=w489:i32)  [unwired: 1 in, 3 out]
          n250 = Less Than 0?(x=w489) -> (x < 0?=w488:bool)
        }
        n251 = for {
          tunnel: w476 -> [w487] mode=indexing
          tunnel: w478 -> [w486]
          tunnel: [w485] -> w477 if=w483
          i -> [w485]
          stop <- w483 stop-if-true
          n252 = Search/Split String(string=w487, search string/char (-)=w486) -> (offset of match=w484:i32)  [unwired: 1 in, 2 out]
          n253 = Greater Or Equal To 0?(x=w484) -> (x >= 0?=w483:bool)
        }
        n254 = Index Array(array=w476, index=w477) -> (element=w475:string)
        n255 = Build Array(w475) -> (w471:string[])
        n256 = property class="Tree (strict)"(reference=w474, error in=w473, "Value"=w471) -> (error out=w472:errorcluster)  [unwired: 1 out]
      }
      frame "API: Set Current CSM" {
        n257 = control-ref of="MainTree"() -> (w500:refnum<vi>)
        n258 = property class="Tree (strict)"(reference=w500) -> (reference out=w498:refnum<vi>, error out=w497:errorcluster, "All Tags"=w494:string[])  [unwired: 1 in]
        n259 = for {
          tunnel: w494 -> [w510] mode=indexing
          tunnel: w493 -> [w507]
          tunnel: [w504] -> w492 if=w503
          i -> [w504]
          stop <- w503 stop-if-true
          n260 = Match Pattern(string=w510, regular expression="/") -> (after substring=w508:string, offset past match=w509:i32)  [unwired: 1 in, 2 out]
          n261 = Equal?(x=w508, y=w507) -> (x = y?=w506:bool)
          n262 = Greater Or Equal To 0?(x=w509) -> (x >= 0?=w505:bool)
          n263 = And(x=w506, y=w505) -> (x .and. y?=w503:bool)
        }
        n264 = Index Array(array=w494, index=w492) -> (element=w499:string)
        n265 = Build Array(w499) -> (w495:string[])
        n266 = property class="Tree (strict)"(reference=w498, error in=w497, "Value"=w495) -> (error out=w496:errorcluster)  [unwired: 1 out]
      }
      frame "---------- Action ----------" {
        n267 = call <vilib>:"Add State(s) to Queue__JKI_lib_State_Machine.vi"("State(s) in (\"\")"=w514) -> ("States Out"=w513:string)  [unwired: 14 in]
      }
      frame "Action: Refresh(CSM mode)" {
        n268 = control-ref of="MainTree"() -> (w522:refnum<vi>)
        n269 = call "build tree table in CSM mode.vi"() -> ("Error Out"=w516:errorcluster, "Type"=w517:string[], "Tree Table"=w518:string[][])  [unwired: 9 in]
        n270 = call "Populate Tree with Delimited Strings_csm.vi"("Default Symbol"=0, "Delimiter"="/", "Items (Delimited)"=w518, "Tree Control"=w522) -> ("error out"=w520:errorcluster, "Tree Control Dup"=w519:refnum<vi>)  [unwired: 5 in, 1 out]
        n271 = property class="Tree"(reference=w519, error in=w520, "RowHdrs[]"=w517) -> ()  [unwired: 2 out]
        n272 = call <vilib>:"Add State(s) to Queue__JKI_lib_State_Machine.vi"("State(s) in (\"\")"=w525) -> ("States Out"=w524:string)  [unwired: 14 in]
      }
      frame "Action: Refresh(CSM-VI mode)" {
        n273 = Bundle By Name(cluster=T6 {"Opton:All-CSM-VIs"=FALSE, "Option:Online Only"=FALSE} ("Option"), "Opton:All-CSM-VIs"="Option:All-CSM-VIs", "Option:Online Only"="Option:Online Only") -> (w528:T6)
        n274 = call "build tree table in CSM-VI mode.vi"("Option"=w528) -> ("Type"=w531:string[], "Tree Table"=w532:string[][])  [unwired: 8 in, 1 out]
        n275 = Bundle By Name(cluster=w534, "Tree.Table"=w532, "Tree.Type"=w531) -> (w533:T10)
        n276 = call <vilib>:"Add State(s) to Queue__JKI_lib_State_Machine.vi"("State(s) in Front (\"\")"="Action: Update Tree" ("State(s) in Front (\"\")"), "State(s) in (\"\")"=w536) -> ("States Out"=w535:string)  [unwired: 13 in]
      }
      frame "Action: Update Online CSMs" {
        n277 = call "Refresh Online CSMs in lvcsm.vi"("Caller"=w539) -> ("error out"=w538:errorcluster, "Array W/ Subset Deleted"=w537:string[])  [unwired: 9 in]
        n278 = Empty Array?(array=w537) -> (empty?=w541:bool)
        n279 = Merge Errors(w538) -> (w542:errorcluster)
        n280 = call-poly "Add State(s) to Queue By BOOL++.vi"("FALSE (\"\")"="Action: Refresh(CSM-VI mode)" ("State(s) in Front (\"\")"), "Condition"=w541, "State Queue (\"\")"=w543) -> ("Remaining States"=w545:string)  [unwired: 8 in]
      }
      frame "Action: Update Tree" {
        n281 = Unbundle By Name(w550) -> ("Tree"=w549:T9)
        n282 = call "Filter Tree Data.vi"("FilterOption"="FilterOption", "Filter"="Filter", "TreeData"=w549) -> ("TreeData 2"=w551:T9)  [unwired: 8 in]
        n283 = Unbundle By Name(w551) -> ("Table"=w547:string[][], "Type"=w546:string[])
        n284 = control-ref of="MainTree"() -> (w557:refnum<vi>)
        n285 = call "Populate Tree with Delimited Strings_csm.vi"("Default Symbol"=0, "Delimiter"="/", "Items (Delimited)"=w547, "Tree Control"=w557) -> ("error out"=w555:errorcluster, "Tree Control Dup"=w554:refnum<vi>)  [unwired: 5 in, 1 out]
        n286 = property class="Tree"(reference=w554, error in=w555, "RowHdrs[]"=w546) -> ()  [unwired: 2 out]
        n287 = call <vilib>:"Add State(s) to Queue__JKI_lib_State_Machine.vi"("State(s) in (\"\")"=w559) -> ("States Out"=w558:string)  [unwired: 14 in]
      }
      frame "Action: Refresh Interface" {
        n288 = control-ref of="MainTree"() -> (w566:refnum<vi>)
        n289 = property class="Tree (strict)"(reference=w566) -> ("Value"=w565:string[])  [unwired: 1 in, 2 out]
        n290 = for {
          tunnel: [w604] -> w573 mode=indexing
          tunnel: w565 -> [w602] mode=indexing
          n291 = Match Pattern(string=w602, regular expression="/") -> (before substring=w601:string)  [unwired: 1 in, 3 out]
          n292 = call "Read CSM States By CSM-VI.vi"("CSM VI"=w601) -> ("Array"=w605:string[])  [unwired: 9 in, 1 out]
          n293 = Bundle("Array"=w605) -> (w604:cluster{"Array":string[]})  [unwired: 1 in]
        }
        n294 = Delete From Array(array=w573, index=0) -> (deleted portion=w570:cluster{"Array":string[]}, array with subset deleted=w571:cluster{"Array":string[]}[])  [unwired: 1 in]
        n295 = Unbundle(w570) -> ("Array"=w569:string[])
        n296 = for {
          tunnel: w571 -> [w597] mode=indexing
          shift-right: [w592] -> w568
          shift-left: w569 -> [w596]
          n297 = Unbundle(w597) -> ("Array"=w595:string[])
          n298 = Build Array (concatenate)(w596, w595) -> (w593:string[])
          n299 = call "_Remove Duplicates Strings.vi"("Input Array"=w593) -> ("Indices of Removed Elements"=w594:i32[])  [unwired: 1 out]
          n300 = for {
            tunnel: w594 -> [w599] mode=indexing
            tunnel: w593 -> [w600]
            tunnel: [w598] -> w592 mode=indexing
            n301 = Index Array(array=w600, index=w599) -> (element=w598:string)
          }
        }
        n302 = local read "FilterOption"() -> (w562:T2)
        n303 = local read "Filter"() -> (w561:string)
        n304 = call "filter CSM States.vi"("Interface-Filter"="Interface-Filter", "Array"=w568) -> ("filtered array"=w563:string[])  [unwired: 9 in]
        n305 = call <vilib>:"Add State(s) to Queue__JKI_lib_State_Machine.vi"("State(s) in (\"\")"=w576) -> ("States Out"=w575:string)  [unwired: 14 in]
        n306 = case shown="\"State\"" w562 {
          tunnel: [w577 w581] -> w564
          tunnel: w563 -> [w577 w580]
          tunnel: w561 -> [_ w579]
          tunnel: "Option:Sync Filter On States" -> [_ w578]
          frame "Name", Default {
          }
          frame "State" {
            n307 = case shown="False" w578 {
              tunnel: [w582 w585] -> w581
              tunnel: w580 -> [w582 w584]
              tunnel: w579 -> [_ w583]
              frame False {
              }
              frame True {
                n308 = for {
                  tunnel: [w588] -> w585 mode=indexing if=w586
                  tunnel: w584 -> [w588] mode=indexing
                  tunnel: w583 -> [w587]
                  n309 = To Lower Case(string=w587) -> (all lower case string=w589:string)
                  n310 = To Lower Case(string=w588) -> (all lower case string=w590:string)
                  n311 = Match Pattern(string=w590, regular expression=w589) -> (offset past match=w591:i32)  [unwired: 1 in, 3 out]
                  n312 = Greater Or Equal To 0?(x=w591) -> (x >= 0?=w586:bool)
                }
              }
            }
          }
        }
        n313 = property on="CSM-States" class="LstBox (strict)"("Item Names"=w564) -> ()  [unwired: 2 in, 2 out]
      }
      frame "Action: Refresh Status List" {
        n314 = control-ref of="MainTree"() -> (w612:refnum<vi>)
        n315 = property class="Tree (strict)"(reference=w612) -> ("Value"=w611:string[])  [unwired: 1 in, 2 out]
        n316 = Index Array(array=w611) -> (element=w610:string)  [unwired: 1 in]
        n317 = Match Pattern(string=w610, regular expression="/") -> (before substring=w608:string)  [unwired: 1 in, 3 out]
        n318 = call "Read CSM Status By CSM-VI.vi"("CSM VI"=w608) -> ("Array 3"=w607:cluster{"Status":string, "InState":string}[])  [unwired: 9 in, 1 out]
        n319 = disable-structure shown="Enabled" {
          disable-tunnel: w607 -> [w618 w623 _]
          disable-tunnel: [w616 w621 _] -> w606
          frame Disabled {
            n320 = for {
              tunnel: w618 -> [w620] mode=indexing
              tunnel: [w619] -> w617 mode=indexing
              n321 = Unbundle(w620) -> ("Status"=w619:string)  [unwired: 1 out]
            }
            n322 = call "_Remove Duplicates Strings.vi"("Input Array"=w617) -> ("Output Array"=w616:string[])  [unwired: 1 out]
          }
          frame Enabled {
            n323 = for {
              tunnel: w623 -> [w627] mode=indexing
              tunnel: [w625] -> w622 mode=indexing
              n324 = Unbundle(w627) -> ("Status"=w626:string, "InState"=w624:string)
              n325 = case shown="\"\"" w624 {
                selector: w624 -> [w629 _]
                tunnel: w626 -> [w631 w632]
                tunnel: [w630 w632] -> w625
                frame Default {
                  n326 = Concatenate Strings(w631, " @ " ("string"), w629) -> (w630:string)
                }
                frame "" {
                }
              }
            }
            n327 = call "_Remove Duplicates Strings.vi"("Input Array"=w622) -> ("Output Array"=w621:string[])  [unwired: 1 out]
          }
          frame Disabled {
          }
        }
        n328 = call <vilib>:"Add State(s) to Queue__JKI_lib_State_Machine.vi"("State(s) in (\"\")"=w615) -> ("States Out"=w614:string)  [unwired: 14 in]
        n329 = property on="CSM-Status" class="LstBox (strict)"("Item Names"=w606) -> ()  [unwired: 2 in, 2 out]
      }
      frame "Action: Refresh Image API" {
        n330 = Match Pattern(string=w637, regular expression="@") -> (before substring=w635:string, after substring=w634:string)  [unwired: 1 in, 2 out]
        n331 = Empty String/Path?(string/path=w634) -> (empty?=w633:bool)
        n332 = case shown="False" w633 {
          tunnel: [w649 _] -> w639
          tunnel: [w648 _] -> w638
          tunnel: w634 -> [w646 _]
          tunnel: w635 -> [w645 _]
          frame False {
            n333 = local read "Zoom Factor"() -> (w642:dbl)
            n334 = control-ref of="Preview"() -> (w644:refnum<vi>)
            n335 = Format Into String(format string="%s@%s", w645, w646) -> (resulting string=w648:string)  [unwired: 2 in, 1 out]
            n336 = call "Update Case Frame to Image.vi"("Zoom Factor"=w642, "Picture Control Reference"=w644, "Type"=enum16{"CSM", "CSM-VI"}."CSM-VI", "State"=w645, "Name"=w646) -> ("Error Out"=w649:errorcluster)  [unwired: 5 in, 1 out]
          }
          frame True {
          }
        }
        "StateInfo@Image" <- w638
      }
      frame "Action: Refresh Image" {
        n337 = control-ref of="CSM-States"() -> (w664:refnum<vi>)
        n338 = property class="LstBox (strict)"(reference=w664) -> ("Item Names"=w665:string[], "Value"=w663:i32[])  [unwired: 1 in, 2 out]
        n339 = control-ref of="MainTree"() -> (w661:refnum<vi>)
        n340 = property class="Tree (strict)"(reference=w661) -> ("Value"=w660:string[])  [unwired: 1 in, 2 out]
        n341 = Index Array(array=w663) -> (element=w662:i32)  [unwired: 1 in]
        n342 = Index Array(array=w660) -> (element=w659:string)  [unwired: 1 in]
        n343 = Match Pattern(string=w659, regular expression="/") -> (before substring=w653:string)  [unwired: 1 in, 3 out]
        n344 = Index Array(array=w665, index=w662) -> (element=w654:string)
        n345 = Concatenate Strings(w654, "@" ("string"), w653) -> (w651:string)
        n346 = call <vilib>:"Build State String with Arguments__JKI_lib_State_Machine.vi"("Arguments (\"\")"=w651, "State"="Action: Refresh Image API") -> ("State with Arguments"=w650:string)  [unwired: 4 in]
        n347 = call <vilib>:"Add State(s) to Queue__jki_lib_state_machine.vi"("State(s) in Front (\"\")"=w650, "State(s) in (\"\")"=w656) -> ("States Out"=w657:string)  [unwired: 13 in]
      }
      frame "Action: Refresh Image2" {
        n348 = control-ref of="CSM-Status"() -> (w671:refnum<vi>)
        n349 = property class="LstBox (strict)"(reference=w671) -> ("Item Names"=w685:string[], "Value"=w684:i32[])  [unwired: 1 in, 2 out]
        n350 = control-ref of="MainTree"() -> (w682:refnum<vi>)
        n351 = property class="Tree (strict)"(reference=w682) -> ("Value"=w681:string[])  [unwired: 1 in, 2 out]
        n352 = Index Array(array=w684) -> (element=w683:i32)  [unwired: 1 in]
        n353 = Index Array(array=w681) -> (element=w680:string)  [unwired: 1 in]
        n354 = Match Pattern(string=w680, regular expression="/") -> (before substring=w675:string)  [unwired: 1 in, 3 out]
        n355 = Index Array(array=w685, index=w683) -> (element=w669:string)
        n356 = Match Pattern(string=w669, regular expression="@") -> (after substring=w668:string)  [unwired: 1 in, 3 out]
        n357 = call <vilib>:"Trim Whitespace.vi"("string"=w668) -> ("trimmed string"=w667:string)  [unwired: 1 in]
        n358 = Concatenate Strings(w667, "@" ("string"), w675) -> (w673:string)
        n359 = call <vilib>:"Build State String with Arguments__JKI_lib_State_Machine.vi"("Arguments (\"\")"=w673, "State"="Action: Refresh Image API") -> ("State with Arguments"=w672:string)  [unwired: 4 in]
        n360 = call <vilib>:"Add State(s) to Queue__jki_lib_state_machine.vi"("State(s) in Front (\"\")"=w672, "State(s) in (\"\")"=w677) -> ("States Out"=w678:string)  [unwired: 13 in]
      }
      frame "Action: Refresh Symbol" {
        n361 = control-ref of="MainTree"() -> (w695:refnum<vi>)
        n362 = property class="Tree (strict)"(reference=w695) -> (reference out=w693:refnum<vi>, "All Tags"=w694:string[], "OwningVI"=w688:refnum<vi>)  [unwired: 1 in, 1 out]
        n363 = call "Defer Panel Updates_csm.vi"("Error In"=errorcluster {"status"=FALSE, "code"=0, "source"=""} ("error out"), "Defer Updates?"=TRUE, "VI Reference (Caller)"=w688) -> ("Error Out"=w691:errorcluster)  [unwired: 7 in, 1 out]
        n364 = for {
          tunnel: w694 -> [w700] mode=indexing
          tunnel: w693 -> [w701]
          shift-right: [w699] -> w687
          shift-left: w691 -> [w698]
          n365 = Match Pattern(string=w700, regular expression="/") -> (before substring=w702:string, offset past match=w704:i32)  [unwired: 1 in, 2 out]
          n366 = Less Than 0?(x=w704) -> (x < 0?=w703:bool)
          n367 = case shown="True" w703 {
            tunnel: w702 -> [_ w721]
            tunnel: w701 -> [w708 w722]
            tunnel: w700 -> [w707 w712]
            tunnel: [w709 w711] -> w699
            tunnel: w698 -> [w709 w710]
            frame False {
              n368 = property class="Tree (strict)"(reference=w708, "Active Item Tag"=w707, "Glyph"=18) -> ()  [unwired: 1 in, 2 out]
            }
            frame True {
              n369 = call "Read CSM-VI Info.vi"("CSM Name"=w721) -> ("Cluster 2"=w720:cluster{"Path":path})  [unwired: 9 in, 1 out]
              n370 = Unbundle By Name(w720) -> ("Path"=w719:path)
              n371 = Path To String(path=w719) -> (string=w718:string)
              n372 = call "lvcsm String to Path.vi"("Common Path"=w718) -> ("Path"=w717:path)  [unwired: 10 in]
              n373 = call "_VI Missing or Broken.vi"("Path"=w717) -> ("Missing Or Broken?"=w716:bool)  [unwired: 10 in]
              n374 = Select(t=2, s=w716, f=26) -> (s? t:f=w713:i32)
              n375 = property class="Tree (strict)"(reference=w722, error in=w710, "Active Item Tag"=w712, "Glyph"=w713) -> (error out=w711:errorcluster)  [unwired: 1 out]
            }
          }
        }
        n376 = call "Defer Panel Updates_csm.vi"("Error In"=w687, "Defer Updates?"=FALSE, "VI Reference (Caller)"=w688) -> ()  [unwired: 7 in, 2 out]
      }
      frame "Action: Change Zoom Factor" {
        n377 = Fract/Exp String To Number(string=w724) -> (number=w723:dbl)  [unwired: 3 in, 1 out]
        n378 = control-ref of="Preview"() -> (w725:refnum<vi>)
        n379 = property class="Pict"(reference=w725, "ZoomFactor"=w723) -> ()  [unwired: 1 in, 2 out]
      }
    }
  }
  n380 = while {
    shift-right: [w739] -> _
    shift-left: enum16{"Idle", "Initialize", "Exit"}."Initialize" -> [w740]
    tunnel: "Name (\"\" to Use Uuid)" -> [w737]
    shift-right: [w735] -> _
    shift-left: w12 -> [w736]
    shift-right: [w733] -> _
    shift-left: -1 -> [w734]
    shift-right: [w732] -> _
    shift-left: _ -> [w731]
    shift-right: [w730] -> _
    shift-left: _ -> [w729]
    stop <- w738 stop-if-true
    n381 = case shown="\"Idle\", Default" w740 {
      tunnel: [enum16{"Idle", "Initialize", "Exit"}."Idle" w767 enum16{"Idle", "Initialize", "Exit"}."Exit"] -> w739
      tunnel: [_ _ TRUE] -> w738
      tunnel: w737 -> [w753 w766 _]
      tunnel: w736 -> [w756 w764 w942]
      tunnel: [w756 w765 w942] -> w735
      tunnel: w734 -> [_ w762 _]
      tunnel: [-1 w763 _] -> w733
      tunnel: [w752 w760 _] -> w732
      tunnel: w731 -> [_ w761 w941]
      tunnel: [w748 w758 w939] -> w730
      tunnel: w729 -> [_ w759 w939]
      frame "Initialize" {
        w741 = T11 {"Horizontal"=0, "Vertical"=0}  # PreviewMouseDownOrigin
        w742 = T11 {"Horizontal"=0, "Vertical"=0}  # PreviewMouseDownCoords
        w743 = FALSE  # PreviewMouseDown
        w749 = FALSE  # your data
        n382 = invoke class="VI" method="FP.Open"() -> (reference out=w745:refnum<vi>, error out=w746:errorcluster)  [unwired: 5 in, 3 out]
        n383 = call "CSM - Wait for Module to Be Alive.vi"("CSM Name"=w753) -> ("CSM Name (Dup)"=w751:string, "error out"=w750:errorcluster)  [unwired: 12 in, 1 out]
        n384 = call "Center Callee in Window Bounds.vi"("Error In"=w746, "Callee VI Refnum (Caller)"=w745, "Block Diagram Window:Window Bounds"="Caller Window Bounds") -> ("Error Out"=w747:errorcluster)  [unwired: 8 in]
        n385 = call "CSM - Module Exit Event.vi"("Error In"=w750, "Name (\"\" to Use UUID) In"=w751) -> ("CSM Exit Event"=w754:refnum<user-event>)  [unwired: 7 in, 2 out]
        n386 = call <vilib>:"Clear Errors.vi"("error in (no error)"=w747) -> ()  [unwired: 5 in, 2 out]
        n387 = register-events(w754) -> (reference out=w752:refnum<event-registration>)  [unwired: 2 in, 1 out]
        n388 = Bundle("your data"=w749, "PreviewMouseDown"=w743, "PreviewMouseDownCoords"=w742, "PreviewMouseDownOrigin"=w741) -> (w748:T12)  [unwired: 1 in]
      }
      frame "Idle", Default {
        n389 = event shown="[7] \"Preview\": Mouse Move" {
          selector: w761 -> [_ _ _ _ _ _ _ _ _ _ _ _ _ _ _ _ _ _ _ _ _ _ _ _ _ _ _ _]
          dyn-events: [_ _ _ _ _ _ _ _ _ _ _ _ _ _ _ _ _ _ _ _ _ _ _ _ _ _ _ _] -> w760
          timeout: w762 -> [_ _ _ _ _ _ _ _ _ _ _ _ _ _ _ _ _ _ _ _ _ _ _ _ _ _ _ _]
          tunnel: [_ enum16{"Idle", "Initialize", "Exit"}."Exit" enum16{"Idle", "Initialize", "Exit"}."Exit" _ _ _ _ _ _ _ _ _ _ _ _ _ _ _ _ _ _ _ _ _ _ _ _ _] -> w767
          tunnel: w766 -> [w769 w781 _ _ _ _ _ _ _ _ _ _ _ _ _ _ _ _ _ _ _ _ _ _ _ _ _ _]
          tunnel: w764 -> [w772 _ w786 w791 w794 w805 w809 w815 w823 w831 w834 w839 w843 w852 w857 w861 w865 w869 w880 w892 w900 w903 w905 w911 w916 w921 w931 w936]
          tunnel: [w770 w780 w786 w790 w795 w805 w809 w815 w824 w831 w835 w840 w844 w852 w858 w862 w866 w870 w880 w893 w900 w903 w906 w912 w917 w922 w931 w937] -> w765
          tunnel: [-1 _ _ 50 _ _ _ _ _ _ _ _ _ _ _ _ _ _ _ 20 _ _ 50 50 _ _ _ _] -> w763
          tunnel: w759 -> [w768 w779 w784 w787 w796 w798 w808 w814 w825 w830 w836 w841 w845 w851 w859 w863 w867 w871 w879 w896 w899 w902 w908 w914 w918 w923 w930 w938]
          tunnel: [w768 w779 w784 w787 w796 w797 w807 w814 w825 w830 w836 w841 w845 w851 w859 w863 w867 w871 w879 w896 w899 w902 w908 w914 w918 w923 w930 w938] -> w758
          event Timeout {
            n390 = event-data() -> ()  [unwired: 1 in, 3 out]
            n391 = call-poly "CSM - Filter JKISM String Queue.vi"("States In"=w772) -> ("States Out"=w771:string)  [unwired: 14 in]
            n392 = call "CSM - Forward UI Operations to CSM.vi"("Name (\"\" to Use UUID)"=w769, "State(s) In (\"\")"=w771) -> ("States Out"=w770:string)  [unwired: 8 in, 1 out]
          }
          event Panel Close? {
            n393 = event-data() -> ()  [unwired: 1 in, 1 out]
            n394 = call "CSM - Forward UI Operations to CSM.vi"("Name (\"\" to Use UUID)"=w781, "State(s) In (\"\")"="Macro: Exit" ("State")) -> ("States Out"=w780:string)  [unwired: 8 in, 1 out]
            n395 = Current VI's Path() -> (path=w778:path)
            n396 = Path To String(path=w778) -> (string=w777:string)
            n397 = Match Pattern(string=w777, regular expression="National Instruments") -> (offset past match=w775:i32)  [unwired: 1 in, 3 out]
            n398 = Less Than 0?(x=w775) -> (x < 0?=w774:bool)
            n399 = event-data("Discard?"=w774) -> ()  [unwired: 1 in, 1 out]
          }
          event User Event {
            n400 = event-data() -> ()  [unwired: 1 in, 1 out]
          }
          event Panel Resize {
            # "Wait 50ms to prevent flood of events"
            n401 = event-data() -> ()  [unwired: 1 in, 3 out]
            n402 = call <vilib>:"Add State(s) to Queue__JKI_lib_State_Machine.vi"("State(s) in (\"\")"=w791, "State(s) at Back (\"\")"="//Panel Size Message to CSM" ("State(s) at Back (\"\")")) -> ("States Out"=w790:string)  [unwired: 13 in]
          }
          event "MainTree": Value Change {
            n403 = event-data() -> ()  [unwired: 1 in, 1 out]
            n404 = call <vilib>:"Add State(s) to Queue__JKI_lib_State_Machine.vi"("State(s) in (\"\")"="Action: Refresh Interface\nAction: Refresh Status List" ("State")) -> ("States Out"=w793:string)  [unwired: 14 in]
            n405 = call <vilib>:"Add State(s) to Queue__JKI_lib_State_Machine.vi"("State(s) in Front (\"\")"=w793, "State(s) in (\"\")"=w794) -> ("States Out"=w795:string)  [unwired: 13 in]
          }
          event "Preview": Mouse Down {
            n406 = event-data() -> ("Button"=w799:u16, "CtlRef"=w800:refnum<vi>, "Coords"=w801:T11)  [unwired: 1 in, 2 out]
            n407 = property on="Property Node" class="Pict"(reference=w800) -> ("Origin"=w802:T5)  [unwired: 1 in, 2 out]
            n408 = Equal?(x=w799, y=u16 1) -> (x = y?=w804:bool)
            n409 = Bundle By Name(cluster=w798, "PreviewMouseDown"=w804, "PreviewMouseDownCoords"=w801, "PreviewMouseDownOrigin"=w802) -> (w797:T12)
          }
          event "Preview": Mouse Up {
            n410 = event-data() -> ()  [unwired: 1 in, 5 out]
            n411 = Bundle By Name(cluster=w808, "PreviewMouseDown"=FALSE) -> (w807:T12)
          }
          event "Preview": Mouse Move {
            n412 = event-data() -> ("Coords"=w810:T11)  [unwired: 1 in, 4 out]
            n413 = Unbundle By Name(w814) -> ("PreviewMouseDown"=w813:bool, "PreviewMouseDownCoords"=w812:T11, "PreviewMouseDownOrigin"=w811:T11)
            n414 = case shown="True" w813 {
              tunnel: w812 -> [_ w818]
              tunnel: w811 -> [_ w820]
              tunnel: w810 -> [_ w819]
              frame False {
              }
              frame True {
                n415 = Subtract(x=w819, y=w818) -> (x-y=w821:T11)
                n416 = Subtract(x=w820, y=w821) -> (x-y=w817:T11)
                n417 = control-ref of="Preview"() -> (w816:refnum<vi>)
                n418 = property on="Property Node" class="Pict"(reference=w816, "Origin"=w817) -> ()  [unwired: 1 in, 2 out]
              }
            }
          }
          event "Refresh", "Option:All-CSM-VIs", "Option:Online Only": Value Change {
            n419 = event-data() -> ()  [unwired: 1 in, 1 out]
            n420 = call <vilib>:"Add State(s) to Queue__JKI_lib_State_Machine.vi"("State(s) in Front (\"\")"="Macro: Refresh UI" ("Init State(\"Macro: Initialize\")"), "State(s) in (\"\")"=w823) -> ("States Out"=w824:string)  [unwired: 13 in]
          }
          event "MainTree": Shortcut Menu Activation? {
            n421 = event-data() -> ("CtlRef"=w826:refnum<vi>, "MenuRef"=w828:refnum<k9>, "Coords"=w827:T11)  [unwired: 1 in]
            n422 = call "Build MainTree Menu.vi"("CtlRef"=w826, "Coords"=w827, "Menu In"=w828) -> ("Discard?"=w829:bool)  [unwired: 8 in]
            n423 = event-data("Discard?"=w829) -> ()  [unwired: 1 in, 1 out]
          }
          event "MainTree": Shortcut Menu Selection (User) {
            n424 = event-data() -> ("ItemTag"=w832:string)  [unwired: 1 in, 7 out]
            n425 = case shown="Default" w832 {
              tunnel: [_ "Macro: Refresh UI" ("State(s) at Back (\"\")")] -> w833
              frame "COPY_CNT_FOLDER_TO_CLIPBOARD", "COPY_FULL_PATH_TO_CLIPBOARD", "EXPLORER_TO_FOLDER_ON_CSMVI", "OPEN_CSMVI_ON_CSM", "OPEN_CSMVI_ON_CSMVI" {
              }
              frame Default {
              }
            }
            n426 = call <vilib>:"Add State(s) to Queue__JKI_lib_State_Machine.vi"("State(s) in Front (\"\")"=w832, "State(s) in (\"\")"=w834, "State(s) at Back (\"\")"=w833) -> ("States Out"=w835:string)  [unwired: 12 in]
          }
          event "Interface-Filter": Value Change {
            n427 = event-data() -> ()  [unwired: 1 in, 6 out]
            n428 = call <vilib>:"Add State(s) to Queue__JKI_lib_State_Machine.vi"("State(s) in Front (\"\")"="Action: Refresh Interface" ("State(s) in Front (\"\")"), "State(s) in (\"\")"=w839) -> ("States Out"=w840:string)  [unwired: 13 in]
          }
          event "Open": Value Change {
            n429 = event-data() -> ()  [unwired: 1 in, 1 out]
            n430 = call <vilib>:"Add State(s) to Queue__JKI_lib_State_Machine.vi"("State(s) in Front (\"\")"="ADD_CSMVI_ON_MAINTREEE" ("Init State(\"Macro: Initialize\")"), "State(s) in (\"\")"=w843) -> ("States Out"=w844:string)  [unwired: 13 in]
          }
          event "CSM-States": Shortcut Menu Activation? {
            n431 = event-data() -> ("CtlRef"=w849:refnum<vi>, "MenuRef"=w850:refnum<k9>, "Coords"=w847:T11)  [unwired: 1 in, 4 out]
            n432 = control-ref of="MainTree"() -> (w846:refnum<vi>)
            n433 = call "Build Interface Menu.vi"("Tree"=w846, "CtlRef"=w849, "Coords"=w847, "Menu In"=w850) -> ("Discard?"=w848:bool)  [unwired: 7 in]
            n434 = event-data("Discard?"=w848) -> ()  [unwired: 1 in, 1 out]
          }
          event "CSM-States": Shortcut Menu Selection (User) {
            n435 = event-data() -> ("ItemTag"=w855:string)  [unwired: 1 in, 7 out]
            n436 = Match Pattern(string=w855, regular expression="#") -> (before substring=w853:string)  [unwired: 1 in, 3 out]
            n437 = call <vilib>:"Add State(s) to Queue__JKI_lib_State_Machine.vi"("State(s) in Front (\"\")"=w853, "State(s) in (\"\")"=w857, "State(s) at Back (\"\")"="" ("State(s) at Back (\"\")")) -> ("States Out"=w858:string)  [unwired: 12 in]
          }
          event "Scan Project": Value Change {
            n438 = event-data() -> ()  [unwired: 1 in, 5 out]
            n439 = call <vilib>:"Add State(s) to Queue__JKI_lib_State_Machine.vi"("State(s) in Front (\"\")"="SCAN_ALL_CSMVI\nMacro: Refresh UI" ("State(s) in Front (\"\")"), "State(s) in (\"\")"=w861) -> ("States Out"=w862:string)  [unwired: 13 in]
          }
          event "CSM-States": Double Click {
            n440 = event-data() -> ()  [unwired: 1 in, 5 out]
            n441 = call <vilib>:"Add State(s) to Queue__JKI_lib_State_Machine.vi"("State(s) in Front (\"\")"="Action: Refresh Image" ("State(s) in Front (\"\")"), "State(s) in (\"\")"=w865) -> ("States Out"=w866:string)  [unwired: 13 in]
          }
          event "CSM-Status": Double Click {
            n442 = event-data() -> ()  [unwired: 1 in, 5 out]
            n443 = call <vilib>:"Add State(s) to Queue__JKI_lib_State_Machine.vi"("State(s) in Front (\"\")"="Action: Refresh Image2" ("State(s) in Front (\"\")"), "State(s) in (\"\")"=w869) -> ("States Out"=w870:string)  [unwired: 13 in]
          }
          event "MainTree": Mouse Move {
            n444 = event-data() -> ("CtlRef"=w878:refnum<vi>, "Coords"=w877:T11)  [unwired: 1 in, 3 out]
            n445 = invoke class="Tree (strict)" method="Point To Row Column"(reference=w878, "Point"=w877) -> ("Tag"=w875:string)  [unwired: 6 in, 7 out]
            n446 = Match Pattern(string=w875, regular expression="/") -> (before substring=w873:string)  [unwired: 1 in, 3 out]
            n447 = feedback-in #1(w873) -> ()
            n448 = feedback #1() -> (w874:string)  [unwired: 1 in]
            n449 = Not Equal?(x=w873, y=w874) -> (x != y?=w872:bool)
            n450 = case shown="True" w872 {
              tunnel: w873 -> [_ w882]
              frame False {
              }
              frame True {
                n451 = call "Read CSM-VI Info.vi"("CSM Name"=w882) -> ("Cluster 2"=w888:cluster{"Path":path})  [unwired: 9 in, 1 out]
                n452 = Unbundle By Name(w888) -> ("Path"=w887:path)
                n453 = Path To String(path=w887) -> (string=w886:string)
                n454 = call "lvcsm String to Path.vi"("Common Path"=w886) -> ("Path"=w885:path)  [unwired: 10 in]
                n455 = Path To String(path=w885) -> (string=w884:string)
                n456 = Concatenate Strings(w882, "  ----  " ("string"), w884) -> (→"String":string)
              }
            }
          }
          event "Zoom Factor": Value Change {
            n457 = event-data() -> ()  [unwired: 1 in, 6 out]
            n458 = Number To Fractional String(number="Zoom Factor") -> (F-format string=w889:string)  [unwired: 3 in]
            n459 = call <vilib>:"Build State String with Arguments__JKI_lib_State_Machine.vi"("Arguments (\"\")"=w889, "State"="Action: Change Zoom Factor" ("State(s) in Front (\"\")")) -> ("State with Arguments"=w891:string)  [unwired: 4 in]
            n460 = call <vilib>:"Add State(s) to Queue__JKI_lib_State_Machine.vi"("State(s) in Front (\"\")"=w891, "State(s) in (\"\")"=w892) -> ("States Out"=w893:string)  [unwired: 13 in]
          }
          event "Zoom Factor", "Option:All-CSM-VIs", "Scan Project", "Preview", "Open", "Interface-Filter", "Play", "Fast Forward", "Fast Reverse", "Skip to Beginning", "Stop", "MainTree", "CSM-States": Mouse Enter {
            n461 = event-data() -> ("CtlRef"=w898:refnum<vi>)  [unwired: 1 in, 3 out]
            n462 = property class="Ctl"(reference=w898) -> ("TipStrip"=w897:string)  [unwired: 1 in, 2 out]
            n463 = local write "String"(w897) -> ()
          }
          event "MainTree", "CSM-States", "Interface-Filter", "Open", "Play", "Stop", "Skip to End", "Skip to Beginning", "Preview", "Fast Reverse", "Fast Forward", "Scan Project", "Option:All-CSM-VIs", "Zoom Factor": Mouse Leave {
            n464 = event-data() -> ()  [unwired: 1 in, 4 out]
            n465 = local write "String"("" ("String")) -> ()
          }
          event "Filter": Value Change {
            n466 = event-data() -> ()  [unwired: 1 in, 5 out]
            n467 = call <vilib>:"Add State(s) to Queue__JKI_lib_State_Machine.vi"("State(s) in Front (\"\")"="Action: Update Tree\nAction: Refresh Symbol" ("State(s) in Front (\"\")"), "State(s) in (\"\")"=w905) -> ("States Out"=w906:string)  [unwired: 13 in]
          }
          event "Reset Filter": Value Change {
            n468 = event-data() -> ()  [unwired: 1 in, 5 out]
            n469 = local write "Filter"("" ("Filter")) -> ()
            n470 = call <vilib>:"Add State(s) to Queue__JKI_lib_State_Machine.vi"("State(s) in Front (\"\")"="Action: Update Tree\nAction: Refresh Symbol" ("State(s) in Front (\"\")"), "State(s) in (\"\")"=w911) -> ("States Out"=w912:string)  [unwired: 13 in]
          }
          event "Refresh lvcsm Cache": Value Change {
            n471 = event-data() -> ()  [unwired: 1 in, 6 out]
            n472 = call <vilib>:"Add State(s) to Queue__JKI_lib_State_Machine.vi"("State(s) in Front (\"\")"="Action: Update Online CSMs\nAction: Refresh Symbol" ("State(s) in Front (\"\")"), "State(s) in (\"\")"=w916) -> ("States Out"=w917:string)  [unwired: 13 in]
          }
          event "Option:Sync Filter On States": Value Change {
            n473 = event-data() -> ()  [unwired: 1 in, 5 out]
            n474 = local read "FilterOption"() -> (w919:T2)
            n475 = case shown="\"State\"" w919 {
              tunnel: [_ "Action: Refresh Interface" ("Init State(\"Macro: Initialize\")")] -> w920
              frame "Name", Default {
              }
              frame "State" {
              }
            }
            n476 = call <vilib>:"Add State(s) to Queue__JKI_lib_State_Machine.vi"("State(s) in Front (\"\")"=w920, "State(s) in (\"\")"=w921) -> ("States Out"=w922:string)  [unwired: 13 in]
          }
          event "CSM-Status": Shortcut Menu Activation? {
            n477 = event-data() -> ("CtlRef"=w925:refnum<vi>, "MenuRef"=w928:refnum<k9>, "Coords"=w929:T11)  [unwired: 1 in, 4 out]
            n478 = control-ref of="MainTree"() -> (w926:refnum<vi>)
            n479 = call "Build Status Menu.vi"("Tree"=w926, "CtlRef"=w925, "Coords"=w929, "Menu In"=w928) -> ("Discard?"=w927:bool)  [unwired: 7 in]
            n480 = event-data("Discard?"=w927) -> ()  [unwired: 1 in, 1 out]
          }
          event "CSM-Status": Shortcut Menu Selection (User) {
            n481 = event-data() -> ("ItemTag"=w934:string)  [unwired: 1 in, 7 out]
            n482 = Match Pattern(string=w934, regular expression="#") -> (before substring=w932:string)  [unwired: 1 in, 3 out]
            n483 = call <vilib>:"Add State(s) to Queue__JKI_lib_State_Machine.vi"("State(s) in Front (\"\")"=w932, "State(s) in (\"\")"=w936, "State(s) at Back (\"\")"="" ("State(s) at Back (\"\")")) -> ("States Out"=w937:string)  [unwired: 12 in]
          }
        }
      }
      frame "Exit" {
        n484 = Unregister For Events(event registration refnum=w941) -> (error out=w940:errorcluster)  [unwired: 1 in]
        n485 = call <vilib>:"Clear Errors.vi"("error in (no error)"=w940) -> ()  [unwired: 5 in, 2 out]
      }
    }
  }
  n486 = control-ref of="Current VI Reference"() -> (w2:refnum<vi>)
  n487 = call "Close FP if in LabVIEW Dir.vi"("VI Refnum"=w2, "Error in"=w1) -> ("Error out"=w3:errorcluster)  [unwired: 9 in]
  n488 = call <vilib>:"Clear Errors.vi"("error in (no error)"=w3) -> ()  [unwired: 5 in, 2 out]
